vi "Main.vi"(11 "Module Admin":refnum<class "Delacor_lib_QMH_Cloneable Module Admin.lvclass">) -> ()   [LabVIEW 2020, in "Data Viewer.lvlib"]
doc: "This template is based off of the Queued Message Handler design pattern and the Queued Message Handler project template that ships with LabVIEW.\n\nThe main difference is that the queue is private to this module and communication between modules is performed via Broadcast and Request events.\n\nRequest events are wrapped in public API methods and are handled in the Event Handling Loop (EHL) of this VI. Any module can register for Broadcast events sent by this module. The EHL generates messages based on user interface actions.\n\nThe Message Handling Loop (MHL) processes messages generated by the EHL, or by other messages. The messages are string values, so new messages can be added easily to the Message Cases case structure in the MHL. Each message cluster can also provide an optional value for Message Data, which is a variant that can be converted to whatever message-specific data is required.\n_____\nBased on DQMH Project Template 7.0.1.1316."
uses:
  Data Viewer.lvlib
  <vilib>/Delacor/Delacor QMH/Libraries/Cloneable Module Admin_class/Delacor_lib_QMH_Cloneable Module Admin.lvclass
  C:/Program Files (x86)/National Instruments/LabVIEW 2020/vi.lib/Delacor/Delacor QMH/Libraries/Module Admin_class/Delacor_lib_QMH_Module Admin.lvclass
  Data Viewer/Legend.ctl
  Data Viewer/Filter Arguments.ctl
  Data Viewer/Filter Type.ctl
  Data Viewer/Filter Method.ctl
  <vilib>/Utility/miscctls.llb/LVPoint32TypeDef.ctl
  Data Viewer/Data Viewer.lvclass
  Data Viewer/Control Reference.ctl
  <vilib>/Delacor/Delacor QMH/Libraries/Cloneable Module Admin_class/Delacor_lib_QMH_Cloneable Module Admin.lvclass/Delacor_lib_QMH_Cloneable Module Admin.ctl
  <vilib>/Delacor/Delacor QMH/Libraries/Message Queue_class/Delacor_lib_QMH_Message Queue.lvclass/Delacor_lib_QMH_Message Queue.ctl
  Draw Plot Argument--cluster.ctl
  Filte Data Argument--cluster.ctl
  Menu Action Argument--cluster.ctl
  Open File Argument--cluster.ctl
  Restore Data Argument--cluster.ctl
  Set YScale Argument--cluster.ctl
  Show Value Argument--cluster.ctl
  Update Curve Color Argument--cluster.ctl
  Update Filter Arguments Argument--cluster.ctl
  Window Resize Argument--cluster.ctl
  Stop Argument--cluster.ctl
  Cut Half Data Argument--cluster.ctl
  Scale List Menu Action Argument--cluster.ctl
  Update Scale List Argument--cluster.ctl
  Initialize Plot List Argument--cluster.ctl
  Load Plot Argument--cluster.ctl
  Unload Plot Argument--cluster.ctl
  Show Hide Scale Argument--cluster.ctl
  Add Default Scale Argument--cluster.ctl
  Update Plot List Argument--cluster.ctl
  Add Virtual Cruve Argument--cluster.ctl
  Edit Curve Argument--cluster.ctl
  <vilib>/Utility/miscctls.llb/LVRectTypeDef.ctl
  <vilib>/Delacor/Delacor QMH/Libraries/Module Admin_class/Delacor_lib_QMH_Module Admin.lvclass/Delacor_lib_QMH_Module Admin.ctl
  Data Viewer/Scale Setting--cluster.ctl
  <vilib>/Delacor/Delacor QMH/Libraries/Cloneable Module Admin_class/Delacor_lib_QMH_Get Module ID.vi
  <vilib>/Delacor/Delacor QMH/Libraries/Message Queue_class/Delacor_lib_QMH_Enqueue Message (Single).vi
  <vilib>/Delacor/Delacor QMH/Libraries/Module Admin_class/Delacor_lib_QMH_Get External Launch.vi
  <vilib>/Delacor/Delacor QMH/Libraries/Message Queue_class/Delacor_lib_QMH_Message Queue.lvclass
panel:
  out "图例":T1
  out "Coords":T2
  in  "restore":bool
  in  "Open File":bool
  out "Plot List Select Index":i32
  in  "filter":bool
  in  "滤波参数":T3={"滤波器类型"=enum."Butterworth滤波器", "滤波方式"=enum."低通", "参数1"=1.0, "参数2"=1.0} {"参数2" format="%.2f"; "参数1" format="%.2f"}
  in  "half":bool
  out "Scale List Select Index":i32
  out "移动显示":string
  out "错误输出":errorcluster
  in  "选项卡控件":enum32{"选项卡 1"}(tab)
  in  "Add Virtual Curve":bool
  in  "坐标轴列表":i32(listbox) caption="Y坐标轴"
  in  "Filter Pane":enum32{"选项卡 1", "选项卡 2"}(tab)
  in  "Draw Plot":bool
  in  "X坐标轴":T6
  in  "曲线列表":T7(array[cluster]) caption="曲线" {"Scale" items=["温度", "湿度"]}
  in  "Simulate EHL Error":bool
  in  "Simulate MHL Error":bool
  out "XY图":cluster{"Time":timestamp[], "Value":dbl[]}[](graph)
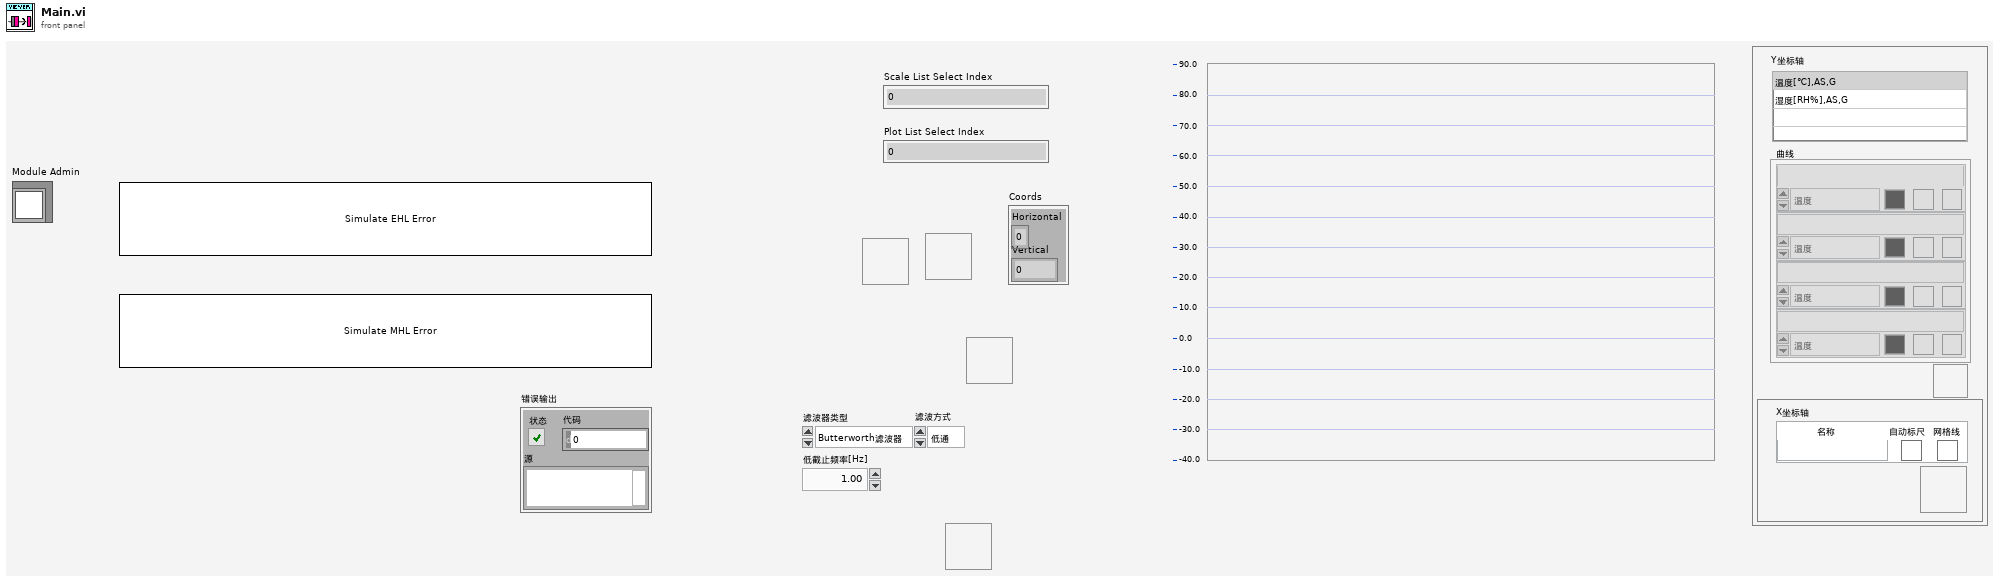
[diagram p1: front panel]
types:
  T1 = typedef "Data Viewer.lvlib/Data Viewer.lvclass/Legend.ctl" = cluster{"颜色":u32, "曲线名称":string}[]
  T2 = typedef "LVPoint32TypeDef.ctl" = cluster{"Horizontal":i32, "Vertical":i32}
  T3 = typedef "Data Viewer.lvlib/Data Viewer.lvclass/Filter Arguments.ctl" = cluster{"滤波器类型":T4, "滤波方式":T5, "参数1":dbl, "参数2":dbl}
  T4 = typedef "Data Viewer.lvlib/Data Viewer.lvclass/Filter Type.ctl" = enum16{"Butterworth滤波器", "中值滤波器"}
  T5 = typedef "Data Viewer.lvlib/Data Viewer.lvclass/Filter Method.ctl" = enum16{"低通", "高通", "带通", "带阻"}
  T6 = cluster{"名称":string, "Auto Scale":bool, "Gird Line":bool}
  T7 = cluster{"Name":string, "Scale":u16, "Color":u32, "Visible":bool, "Peak Line":bool}[]
  T8 = enum8{"Enabled", "Disabled", "Disabled and Grayed Out"}
  T9 = typedef "Data Viewer.lvlib/Data Viewer.lvclass/Control Reference.ctl" = cluster{"rVI":refnum<vi>, "r窗格":refnum<vi>, "rXY图":refnum<vi>, "r选项卡控件":refnum<vi>, "r图例":refnum<vi>, "r移动显示":refnum<vi>, "r滤波参数":refnum<vi>, "rFilter Pane ":refnum<vi>, "r坐标轴列表":refnum<vi>, "rAdd按钮":refnum<vi>, "r曲线列表":refnum<vi>}
  T10 = typedef "Data Viewer.lvlib/Request Events--cluster.ctl" = cluster{"Stop Module":refnum<user-event>, "Show Panel":refnum<user-event>, "Hide Panel":refnum<user-event>, "Show Diagram":refnum<user-event>, "Get Module Execution Status":refnum<user-event>, "Private":cluster{"Window Resize":refnum<user-event>, "Open File":refnum<user-event>, "Draw Plot":refnum<user-event>, "Set YScale":refnum<user-event>, "Update Curve Color":refnum<user-event>, "Show Value":refnum<user-event>, "Menu Action":refnum<user-event>, "Update Filter Arguments":refnum<user-event>, "Filte Data":refnum<user-event>, "Restore Data":refnum<user-event>, "Cut Half Data":refnum<user-event>, "Select Point":refnum<user-event>, "Open Linear Measurement":refnum<user-event>, "Linear Measurement Close":refnum<user-event>}, "Scale List Menu Action":refnum<user-event>, "Private.Update Scale List":refnum<user-event>, "Private.Initialize Plot List":refnum<user-event>, "Private.Load Plot":refnum<user-event>, "Private.Unload Plot":refnum<user-event>, "Show Hide Scale":refnum<user-event>, "Private.Add Default Scale":refnum<user-event>, "Private.Update Plot List":refnum<user-event>, "Private.Add Virtual Cruve":refnum<user-event>, "Private.Edit Curve":refnum<user-event>}
  T11 = typedef "Data Viewer.lvlib/Draw Plot Argument--cluster.ctl" = cluster{"Module ID":i32, "布尔":bool}
  T12 = typedef "Data Viewer.lvlib/Filte Data Argument--cluster.ctl" = cluster{"Module ID":i32, "布尔":bool}
  T13 = typedef "Data Viewer.lvlib/Menu Action Argument--cluster.ctl" = cluster{"Module ID":i32, "项标识符":string}
  T14 = typedef "Data Viewer.lvlib/Open File Argument--cluster.ctl" = cluster{"Module ID":i32, "布尔":bool}
  T15 = typedef "Data Viewer.lvlib/Restore Data Argument--cluster.ctl" = cluster{"Module ID":i32, "布尔":bool}
  T16 = typedef "Data Viewer.lvlib/Set YScale Argument--cluster.ctl" = cluster{"Module ID":i32, "布尔":bool}
  T17 = typedef "Data Viewer.lvlib/Show Value Argument--cluster.ctl" = cluster{"Module ID":i32, "坐标":T2}
  T18 = typedef "Data Viewer.lvlib/Update Curve Color Argument--cluster.ctl" = cluster{"Module ID":i32, "布尔":bool}
  T19 = typedef "Data Viewer.lvlib/Update Filter Arguments Argument--cluster.ctl" = cluster{"Module ID":i32, "布尔":bool}
  T20 = typedef "Data Viewer.lvlib/Window Resize Argument--cluster.ctl" = cluster{"Module ID":i32, "布尔":bool}
  T21 = enum32{"invalid lock state", "Not Locked", "Locked (No Password)", "Password-protected"}
  T22 = typedef "Data Viewer.lvlib/Stop Argument--cluster.ctl" = cluster{"Module ID":i32, "Origin":string, "Exit via Stop Module Req?":bool, "Wait for Module to stop?":bool}
  T23 = typedef "Data Viewer.lvlib/Cut Half Data Argument--cluster.ctl" = cluster{"Module ID":i32, "布尔":bool}
  T24 = typedef "Data Viewer.lvlib/Scale List Menu Action Argument--cluster.ctl" = cluster{"Module ID":i32, "ItemTag ":string, "Scale Index":i32}
  T25 = typedef "Data Viewer.lvlib/Update Scale List Argument--cluster.ctl" = cluster{"Module ID":i32, "Boolean":bool}
  T26 = typedef "Data Viewer.lvlib/Initialize Plot List Argument--cluster.ctl" = cluster{"Module ID":i32, "Boolean":bool}
  T27 = typedef "Data Viewer.lvlib/Load Plot Argument--cluster.ctl" = cluster{"Module ID":i32, "Plot Index":i32}
  T28 = typedef "Data Viewer.lvlib/Unload Plot Argument--cluster.ctl" = cluster{"Module ID":i32, "Plot Index":i32}
  T29 = typedef "Data Viewer.lvlib/Show Hide Scale Argument--cluster.ctl" = cluster{"Module ID":i32, "Scale Index":i32, "Visible":bool}
  T30 = typedef "Data Viewer.lvlib/Add Default Scale Argument--cluster.ctl" = cluster{"Module ID":i32, "Boolean":bool}
  T31 = typedef "Data Viewer.lvlib/Update Plot List Argument--cluster.ctl" = cluster{"Module ID":i32, "曲线列表":cluster{"Name":string, "Scale":u16, "Color":u32, "Visible":bool, "Peak Line":bool}[]}
  T32 = typedef "Data Viewer.lvlib/Add Virtual Cruve Argument--cluster.ctl" = cluster{"Module ID":i32, "Boolean":bool}
  T33 = typedef "Data Viewer.lvlib/Edit Curve Argument--cluster.ctl" = cluster{"Module ID":i32, "Plot Index":i32}
  T34 = typedef "LVRectTypeDef.ctl" = cluster{"Left":i16, "Top":i16, "Right":i16, "Bottom":i16}
  T35 = enum32{"Invalid", "Standard", "Closed", "Hidden", "Minimized", "Maximized"}
  T36 = cluster{"Name":string, "Scale":u16, "Color":u32, "Visible":bool, "Peak LIne":bool}
  T37 = cluster{"Name":string, "Scale":u16, "Color":u32, "Visible":bool, "Peak Line":bool}
  T38 = typedef "Data Viewer.lvlib/Data Viewer.lvclass/Scale Setting--cluster.ctl" = cluster{"Name":string, "Unit":string, "Color":u32, "Auto Scale":bool, "Scale Min":dbl, "Scale Max":dbl, "Scale Interval":dbl, "Show Gird":bool, "Log":bool}
  T39 = enum32{"invalid app kind", "Development System", "Run Time System", "Student Edition", "Embedded LabVIEW", "Evaluation", "Custom"}
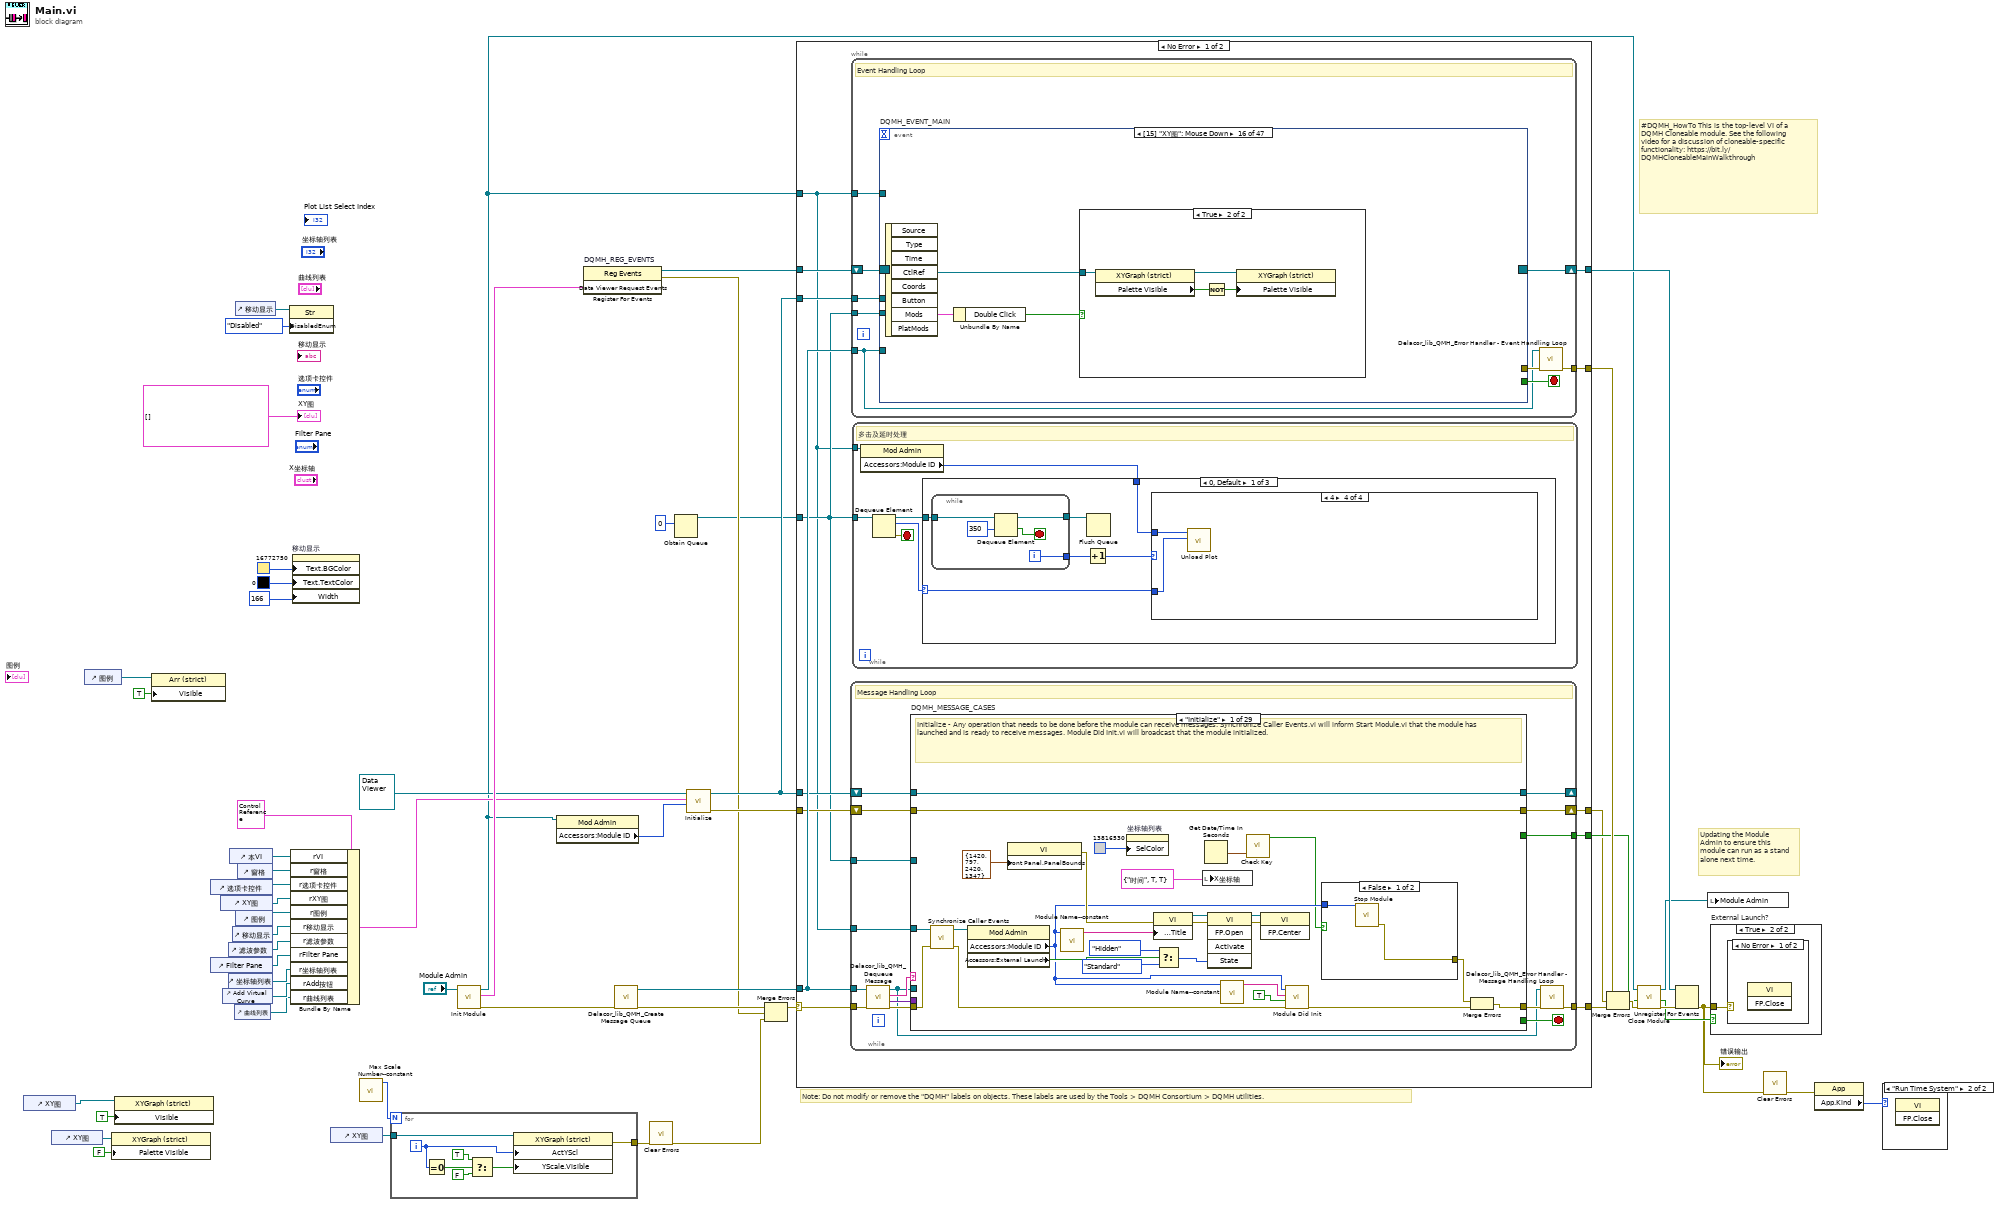
[diagram p0: block diagram]
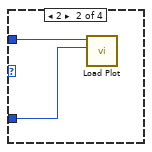
[diagram p4: hidden frame]
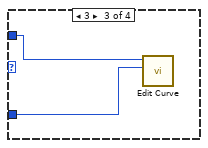
[diagram p5: hidden frame]
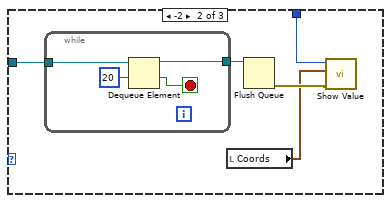
[diagram p6: hidden frame]
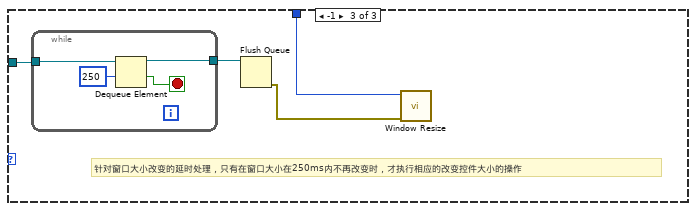
[diagram p7: hidden frame]
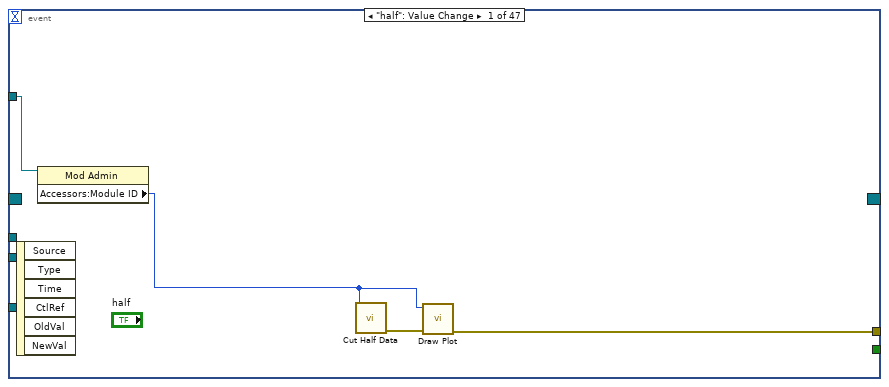
[diagram p8: hidden frame]
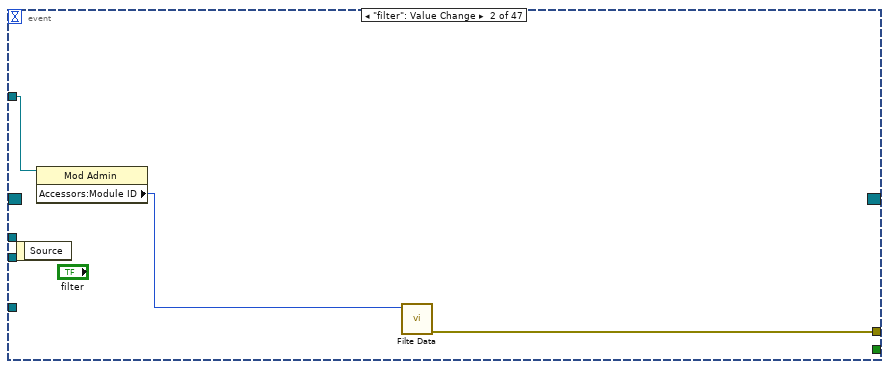
[diagram p9: hidden frame]
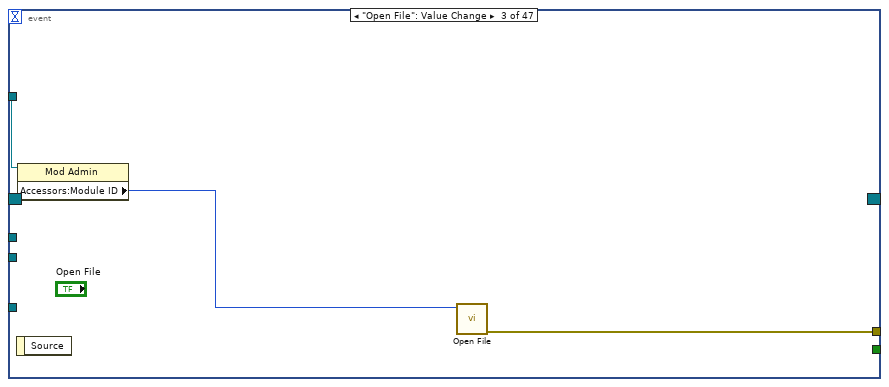
[diagram p10: hidden frame]
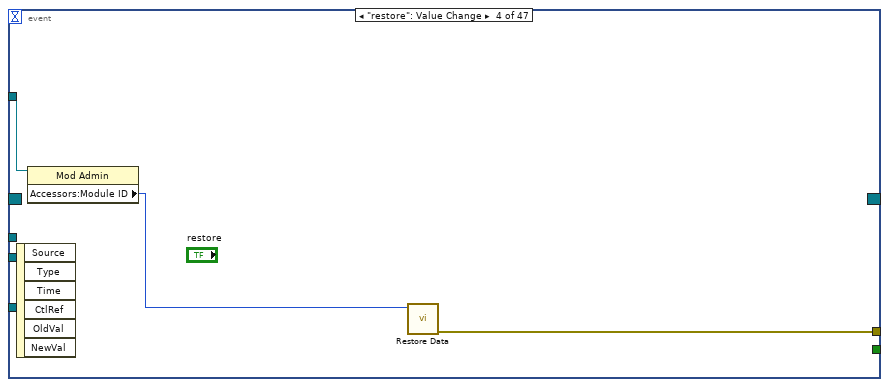
[diagram p11: hidden frame]
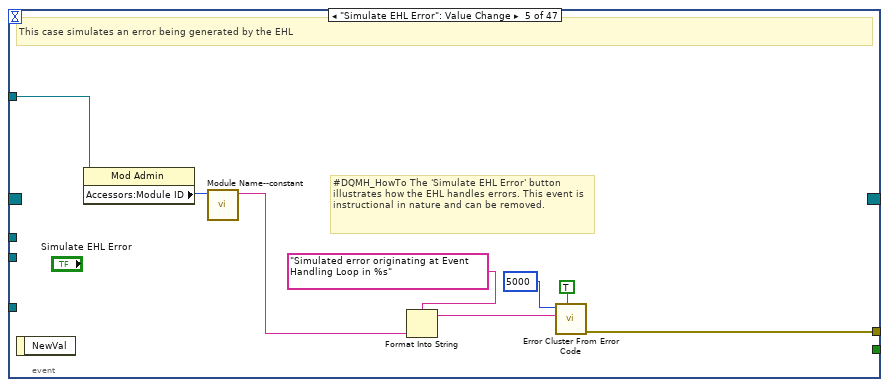
[diagram p12: hidden frame]
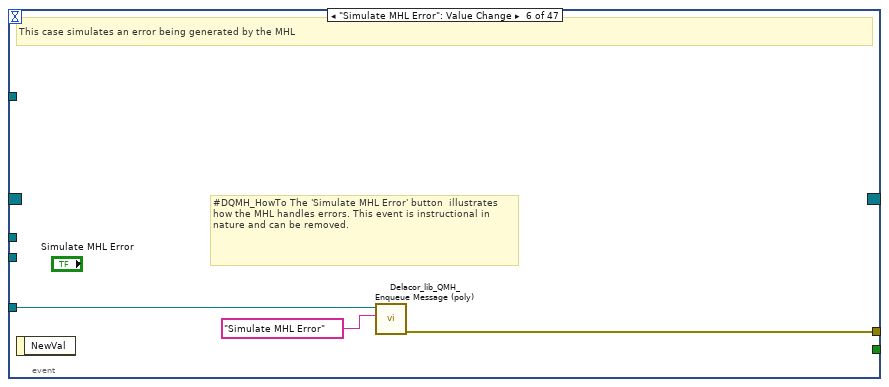
[diagram p13: hidden frame]
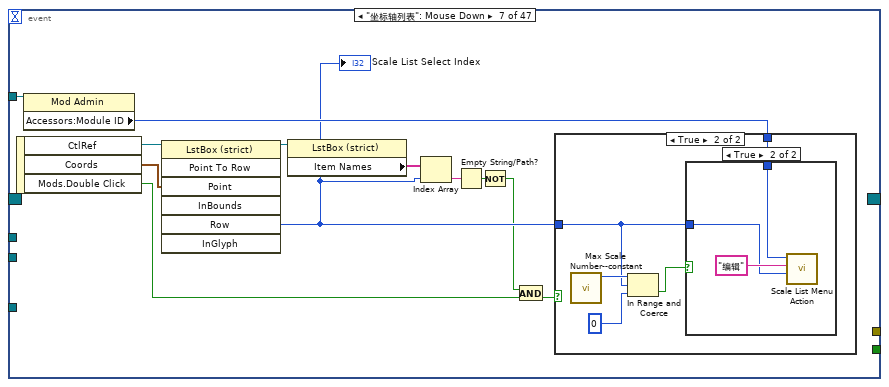
[diagram p14: hidden frame]
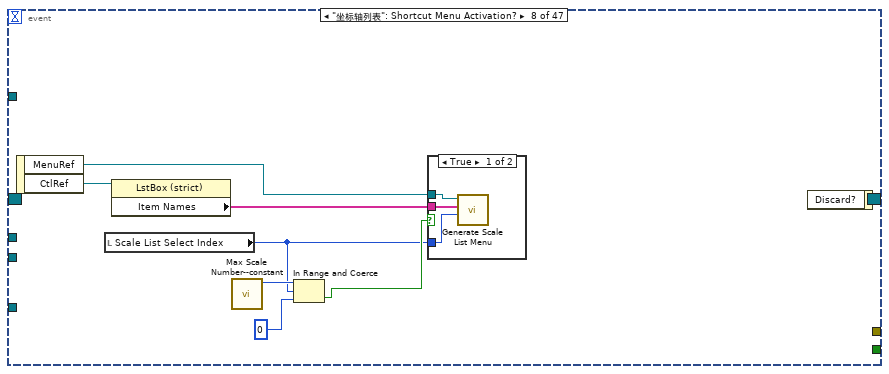
[diagram p17: hidden frame]
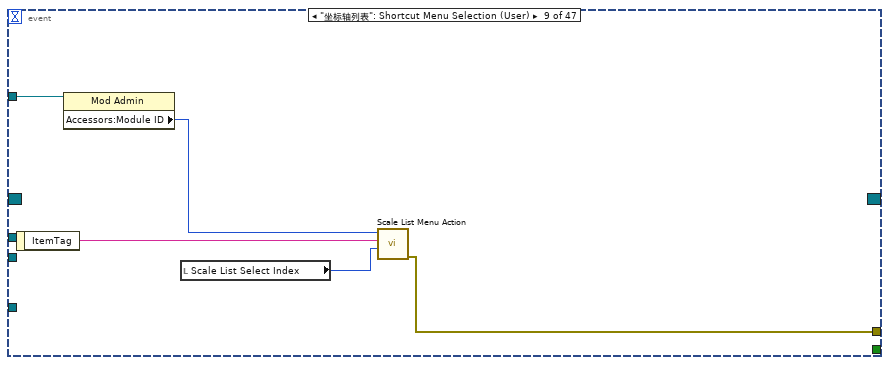
[diagram p19: hidden frame]
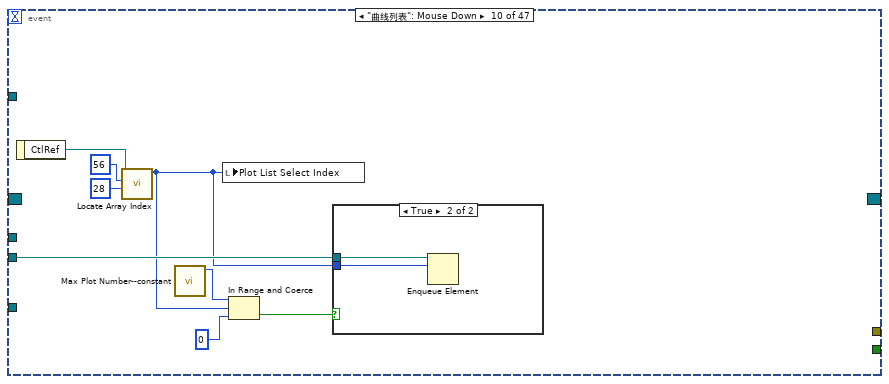
[diagram p20: hidden frame]
diagram:
  # "#DQMH_HowTo This is the top-level VI of a DQMH Cloneable module. See the following video for a discussion of cloneable-specific functionality: https://bit.ly/DQMHCloneableMainWalkthrough"
  # "Note: Do not modify or remove the \"DQMH\" labels on objects. These labels are used by the Tools > DQMH Consortium > DQMH utilities."
  # "Updating the Module Admin to ensure this module can run as a stand alone next time."
  n1 = control-ref of="XY图"() -> (w18:refnum<vi>)
  n2 = control-ref of="XY图"() -> (w2:refnum<vi>)
  n3 = control-ref of="图例"() -> (w4:refnum<vi>)
  n4 = property class="XYGraph (strict)"(reference=w2, "Palette Visible"=FALSE ("Palette:Visible")) -> ()  [unwired: 1 in, 2 out]
  n5 = property class="XYGraph (strict)"(reference=w18, "Visible"=TRUE) -> ()  [unwired: 1 in, 2 out]
  n6 = property class="Arr (strict)"(reference=w4, "Visible"=TRUE) -> ()  [unwired: 1 in, 2 out]
  n7 = control-ref of="选项卡控件"() -> (w34:refnum<vi>)
  n8 = control-ref of="Filter Pane"() -> (w30:refnum<vi>)
  n9 = control-ref of="XY图"() -> (w13:refnum<vi>)
  n10 = control-ref of="Add Virtual Curve"() -> (w6:refnum<vi>)
  n11 = control-ref of="滤波参数"() -> (w29:refnum<vi>)
  n12 = control-ref of="坐标轴列表"() -> (w23:refnum<vi>)
  n13 = control-ref of="本VI"() -> (w37:refnum<vi>)
  n14 = control-ref of="移动显示"() -> (w32:refnum<vi>)
  n15 = control-ref of="曲线列表"() -> (w5:refnum<vi>)
  n16 = control-ref of="移动显示"() -> (w28:refnum<vi>)
  n17 = control-ref of="图例"() -> (w33:refnum<vi>)
  n18 = control-ref of="窗格"() -> (w36:refnum<vi>)
  n19 = property class="Str"(reference=w28, "DisabledEnum"=T8."Disabled" ("禁用")) -> ()  [unwired: 1 in, 2 out]
  n20 = Bundle By Name(cluster=T9 {"rVI"=refnum, "r窗格"=refnum, "rXY图"=refnum, "r选项卡控件"=refnum, "r图例"=refnum, "r移动显示"=refnum, "r滤波参数"=refnum, "rFilter Pane "=refnum, "r坐标轴列表"=refnum, "rAdd按钮"=refnum, "r曲线列表"=refnum} ("Reference"), "rVI"=w37, "r窗格"=w36, "r选项卡控件"=w34, "rXY图"=w13, "r图例"=w33, "r移动显示"=w32, "r滤波参数"=w29, "rFilter Pane"=w30, "r坐标轴列表"=w23, "rAdd按钮"=w6, "r曲线列表"=w5) -> (w38:T9)
  n21 = property on="移动显示" class="Str"("Text.BGColor"=u32 16772750 ("Text.Text Colors:BG Color"), "Text.TextColor"=u32 0 ("Text.Text Colors:Text Color"), "Width"=u32 166 ("Size:Width")) -> ()  [unwired: 2 in, 2 out]
  n22 = control-ref of="XY图"() -> (w19:refnum<vi>)
  n23 = call "Max Scale Number--constant.vi"() -> ("Max Scale Number"=w20:i32)  [unwired: 11 in]
  n24 = for {
    N: w20 -> [_]
    tunnel: w19 -> [w63]
    tunnel: [w58] -> w16
    i -> [w62]
    n25 = Equal To 0?(x=w62) -> (x = 0?=w61:bool)
    n26 = Select(t=TRUE ("Visible"), s=w61, f=FALSE ("Visible")) -> (s? t:f=w57:bool)
    n27 = property class="XYGraph (strict)"(reference=w63, "ActYScl"=w62, "YScale.Visible"=w57) -> (error out=w58:errorcluster)  [unwired: 1 in, 1 out]
  }
  n28 = call "Init Module.vi"("Cloneable Module Admin in"="Module Admin") -> ("error out"=w53:errorcluster, "Data Viewer Request Events"=w47:T10, "Cloneable Module Admin out"=w25:refnum<class "Delacor_lib_QMH_Cloneable Module Admin.lvclass">)  [unwired: 7 in, 1 out]
  n29 = property class="Mod Admin"(reference=w25) -> ("Accessors:Module ID"=w24:i32)  [unwired: 1 in, 2 out]
  n30 = register-events "DQMH_REG_EVENTS"(w47) -> (reference out=w48:refnum<event-registration>, error out=w26:errorcluster)  [unwired: 2 in]
  n31 = call <vilib>:"Delacor_lib_QMH_Create Message Queue.vi"("error in"=w53) -> ("error out"=w51:errorcluster, "Message Queue"=w46:refnum<class "Delacor_lib_QMH_Message Queue.lvclass">)  [unwired: 9 in]
  n32 = call <vilib>:"Clear Errors.vi"("error in (no error)"=w16) -> ("error out"=w15:errorcluster)  [unwired: 5 in, 1 out]
  n33 = Obtain Queue(element data type=0) -> (queue out=w22:refnum<queue>)  [unwired: 4 in, 2 out]
  n34 = call "Initialize.vi"("Module ID"=w24, "Reference"=w38, "Data Viewer 输入"=refnum<class "Data Viewer.lvclass"> refnum ("DataSave.lvlib:Data Viewer.lvlib:Data Viewer.lvclass")) -> ("error out"=w40:errorcluster, "Data Viewer 输出"=w31:refnum<class "Data Viewer.lvclass">)  [unwired: 7 in]
  n35 = Merge Errors(w51, w26, w15) -> (w50:errorcluster)
  n36 = case shown="No Error" w50 {
    selector: w50 -> [w74 w947]
    tunnel: [w76 w946] -> w54
    tunnel: [w73 w945] -> w49
    tunnel: w48 -> [w72 w945]
    tunnel: w46 -> [w71 w938]
    tunnel: [w75 _] -> w55
    tunnel: w25 -> [w64 w941]
    tunnel: [w70 _] -> w43
    tunnel: w31 -> [w69 _]
    tunnel: w40 -> [w68 _]
    tunnel: [w67 _] -> w35
    tunnel: w31 -> [w66 _]
    tunnel: w22 -> [w65 _]
    frame No Error {
      n37 = while {
        tunnel: w71 -> [w557]
        shift-right: [w564] -> _
        shift-left: w69 -> [w565]
        tunnel: w74 -> [w568]
        tunnel: [w566] -> w76
        tunnel: w64 -> [w559]
        tunnel: [w558] -> w70
        shift-right: [w556] -> w67
        shift-left: w68 -> [w555]
        tunnel: w65 -> [w554]
        stop <- w563 stop-if-true
        # "Message Handling Loop"
        n38 = call-dynamic "Delacor_lib_QMH_Dequeue Message.vi"("error in"=w568, "Message Queue in"=w557) -> ("error out"=w567:errorcluster, "Message Data"=w561:variant, "Message"=w562:string, "Message Queue out"=w560:refnum<class "Delacor_lib_QMH_Message Queue.lvclass">)  [unwired: 6 in]
        n39 = case "DQMH_MESSAGE_CASES" shown="\"Initialize\"" w562 {
          selector: w562 -> [_ _ _ _ _ _ _ _ _ _ _ _ _ _ _ _ _ _ _ _ _ _ _ _ _ _ _ _ w927]
          tunnel: w560 -> [_ _ _ _ _ _ _ _ _ _ _ _ _ _ _ _ _ _ _ _ _ _ _ _ _ w875 _ w918 _]
          tunnel: w567 -> [w594 w606 w615 w628 w641 w650 w659 w669 w679 w688 w699 w709 w718 w730 w741 w762 w777 w804 w818 w830 w845 w854 w864 w868 w871 w884 w902 w924 w936]
          tunnel: [w578 w606 w614 w619 w632 w648 w658 w668 w678 w687 w698 w708 w717 w729 w740 w745 w776 w803 w816 w829 w844 w853 w863 w867 w871 w880 w901 w919 w937] -> w569
          tunnel: w565 -> [w582 w605 w610 w623 w640 w649 w654 w663 w674 w683 w694 w704 w711 w725 w736 w751 w772 w799 w817 w825 w840 w849 w859 w866 w870 w879 w899 w908 w934]
          tunnel: [w582 w605 w609 w621 w635 w644 w653 w662 w673 w682 w692 w700 w710 w724 w734 w749 w771 w798 w817 w824 w839 w847 w858 w866 w870 w879 w899 w906 w934] -> w564
          tunnel: [_ _ _ _ _ _ _ _ _ _ _ _ _ _ _ _ _ _ _ _ _ _ _ _ _ _ _ w917 _] -> w563
          tunnel: w561 -> [_ _ w613 w626 w638 w647 w657 w667 w677 w686 w697 w707 w716 w728 w739 w760 w775 w802 w815 w828 w843 w852 w862 _ _ w878 _ w915 _]
          tunnel: w559 -> [w584 _ _ _ _ _ _ _ _ _ _ _ _ _ _ _ _ _ _ _ _ _ _ _ _ w877 w897 w910 w933]
          tunnel: [_ _ _ _ _ _ _ _ _ _ _ _ _ _ _ _ _ _ _ _ _ _ _ _ _ _ _ w913 _] -> w558
          tunnel: [w581 w604 w607 w620 w630 w642 w651 w660 w672 w680 w689 w701 w712 w723 w733 w748 w769 w796 w812 w822 w837 w846 w856 w865 w869 w872 w891 w905 w925] -> w556
          tunnel: w555 -> [w581 w604 w608 w622 w634 w643 w652 w661 w671 w681 w691 w702 w713 w722 w735 w750 w770 w797 w812 w821 w838 w848 w857 w865 w869 w872 w891 w907 w925]
          tunnel: w554 -> [_ _ _ _ _ _ _ _ _ _ _ _ _ _ _ _ _ _ _ _ _ _ _ _ _ _ _ w904 _]
          frame "Initialize" {
            # "Initialize - Any operation that needs to be done before the module can receive messages. Synchronize Caller Events.vi will inform Start Module.vi that the module has launched and is ready to receive messages. Module Did Init.vi will broadcast that the module initialized."
            n40 = call "Synchronize Caller Events.vi"("error in"=w594, "Module Admin"=w584) -> ("error out"=w593:errorcluster, "Module Admin out"=w583:refnum<class "Delacor_lib_QMH_Cloneable Module Admin.lvclass">)  [unwired: 8 in]
            n41 = property on="Property Node" class="Mod Admin"(reference=w583) -> ("Accessors:Module ID"=w573:i32, "Accessors:External Launch"=w585:bool)  [unwired: 1 in, 2 out]
            n42 = property on="Property Node" class="VI"("Front Panel.PanelBounds"=T34 {"Left"=1420, "Top"=797, "Right"=2420, "Bottom"=1347} ("前面板窗口:前面板边界")) -> (error out=w576:errorcluster)  [unwired: 2 in, 1 out]
            n43 = call "Module Name--constant.vi"("Module ID"=w573) -> ("Module Name"=w580:string)  [unwired: 10 in]
            n44 = property on="坐标轴列表" class="LstBox (strict)"("SelColor"=u32 13816530 ("Selection Color")) -> ()  [unwired: 2 in, 2 out]
            n45 = property on="Property Node" class="VI"(error in=w576, "Front Panel.Title"=w580) -> (reference out=w592:refnum<vi>, error out=w596:errorcluster)  [unwired: 1 in]
            n46 = Select(t=T35."Hidden" ("State"), s=w585, f=T35."Standard" ("State")) -> (s? t:f=w588:T35)
            n47 = local write "X坐标轴"(T6 {"名称"="时间", "Auto Scale"=TRUE, "Gird Line"=TRUE} ("X坐标轴")) -> ()
            n48 = Get Date/Time In Seconds() -> (seconds since 1Jan1904=w570:timestamp)
            n49 = invoke on="Invoke Node" class="VI" method="FP.Open"(reference=w592, error in=w596, "State"=w588) -> (reference out=w591:refnum<vi>, error out=w595:errorcluster)  [unwired: 2 in, 3 out]
            n50 = call "Module Name--constant.vi"("Module ID"=w573) -> ("Module Name"=w586:string)  [unwired: 10 in]
            n51 = call "Check Key.vi"("current time"=w570) -> ("Valid?"=w571:bool)  [unwired: 10 in]
            n52 = invoke on="Invoke Node" class="VI" method="FP.Center"(reference=w591, error in=w595) -> ()  [unwired: 1 in, 3 out]
            n53 = call "Module Did Init.vi"("error in"=w593, "Initialized?"=TRUE, "Origin"=w586, "Module ID"=w573) -> ("error out"=w579:errorcluster)  [unwired: 7 in]
            n54 = case shown="False" w571 {
              tunnel: [w597 w600] -> w574
              tunnel: w573 -> [w598 w599]
              frame False {
                n55 = call "Stop Module.vi"("Module ID"=w598) -> ("error out"=w597:errorcluster)  [unwired: 10 in]
              }
              frame True {
                n56 = call "Update Filter Arguments.vi"("Module ID"=w599) -> ("error out"=w603:errorcluster)  [unwired: 10 in]
                n57 = call "Window Resize.vi"("error in"=w603, "Module ID"=w599) -> ("error out"=w602:errorcluster)  [unwired: 9 in]
                n58 = call "Initialize Plot List.vi"("error in"=w602, "Module ID"=w599) -> ("error out"=w601:errorcluster)  [unwired: 9 in]
                n59 = call "Add Default Scale.vi"("error in"=w601, "Module ID"=w599) -> ("error out"=w600:errorcluster)  [unwired: 9 in]
              }
            }
            n60 = Merge Errors(w574, w579) -> (w578:errorcluster)
          }
          frame "---Module Specific---" {
            # "Separator -- The following cases handle messages specific to this Module."
          }
          frame "Window Resize" {
            n61 = Variant To Data(error in=w615, type=T20 {"Module ID"=-1, "布尔"=FALSE} ("Window Resize Argument"), Variant=w613) -> (data=w611:T20, error out=w614:errorcluster)
            n62 = Unbundle By Name(w611) -> ()  [unwired: 2 out]
            n63 = call "Resize Panes.vi"("error in (no error)"=w608, "Data Viewer 输入"=w610) -> ("error out"=w607:errorcluster, "Data Viewer 输出"=w609:refnum<class "Data Viewer.lvclass">)  [unwired: 8 in]
          }
          frame "Open File" {
            n64 = Variant To Data(error in=w628, type=T14 {"Module ID"=-1, "布尔"=FALSE} ("Open File Argument"), Variant=w626) -> (data=w624:T14, error out=w627:errorcluster)
            n65 = Unbundle By Name(w624) -> ("Module ID"=w616:i32)  [unwired: 1 out]
            n66 = call "Set YScale.vi"("Module ID"=w616) -> ("error out"=w617:errorcluster)  [unwired: 10 in]
            n67 = call "Open File.vi"("error in (no error)"=w622, "Data Viewer 输入"=w623) -> ("error out"=w620:errorcluster, "Data Viewer 输出"=w621:refnum<class "Data Viewer.lvclass">)  [unwired: 8 in]
            n68 = call "Draw Plot.vi"("error in"=w617, "Module ID"=w616) -> ("error out"=w618:errorcluster)  [unwired: 9 in]
            n69 = Merge Errors(w618, w627) -> (w619:errorcluster)
          }
          frame "Draw Plot" {
            n70 = Variant To Data(error in=w641, type=T11 {"Module ID"=-1, "布尔"=FALSE} ("Draw Plot Argument"), Variant=w638) -> (data=w636:T11, error out=w639:errorcluster)
            n71 = Unbundle By Name(w636) -> ("Module ID"=w633:i32)  [unwired: 1 out]
            n72 = local read "X坐标轴"() -> (w629:T6)
            n73 = call "Draw Plot.vi"("error in (no error)"=w634, "X坐标轴"=w629, "Data Viewer 输入"=w640) -> ("error out"=w630:errorcluster, "Data Viewer 输出"=w635:refnum<class "Data Viewer.lvclass">)  [unwired: 7 in]
            n74 = call "Window Resize.vi"("error in"=w630, "Module ID"=w633) -> ("error out"=w631:errorcluster)  [unwired: 9 in]
            n75 = Merge Errors(w631, w639) -> (w632:errorcluster)
          }
          frame "Set YScale" {
            n76 = Variant To Data(error in=w650, type=T16 {"Module ID"=-1, "布尔"=FALSE} ("Set YScale Argument"), Variant=w647) -> (data=w645:T16, error out=w648:errorcluster)
            n77 = Unbundle By Name(w645) -> ()  [unwired: 2 out]
            n78 = call "Set YScale.vi"("error in (no error)"=w643, "Data Viewer 输入"=w649) -> ("error out"=w642:errorcluster, "Data Viewer 输出"=w644:refnum<class "Data Viewer.lvclass">)  [unwired: 8 in]
          }
          frame "Update Curve Color" {
            n79 = Variant To Data(error in=w659, type=T18 {"Module ID"=-1, "布尔"=FALSE} ("Update Curve Color Argument"), Variant=w657) -> (data=w655:T18, error out=w658:errorcluster)
            n80 = Unbundle By Name(w655) -> ()  [unwired: 2 out]
            n81 = call "Update Plot Color.vi"("error in (no error)"=w652, "Data Viewer 输入"=w654) -> ("error out"=w651:errorcluster, "Data Viewer 输出"=w653:refnum<class "Data Viewer.lvclass">)  [unwired: 8 in]
          }
          frame "Show Value" {
            n82 = Variant To Data(error in=w669, type=T17 {"Module ID"=-1, "坐标"={"Horizontal"=0, "Vertical"=0}} ("Show Value Argument"), Variant=w667) -> (data=w665:T17, error out=w668:errorcluster)
            n83 = Unbundle By Name(w665) -> ("坐标"=w664:T2)  [unwired: 1 out]
            n84 = call "Show Value.vi"("error in (no error)"=w661, "Coords"=w664, "Data Viewer 输入"=w663) -> ("error out"=w660:errorcluster, "Data Viewer 输出"=w662:refnum<class "Data Viewer.lvclass">)  [unwired: 6 in, 1 out]
          }
          frame "Menu Action" {
            n85 = Variant To Data(error in=w679, type=T13 {"Module ID"=-1, "项标识符"=""} ("Menu Action Argument"), Variant=w677) -> (data=w675:T13, error out=w678:errorcluster)
            n86 = Unbundle By Name(w675) -> ("项标识符"=w670:string)  [unwired: 1 out]
            n87 = call "Menu Action.vi"("error in (no error)"=w671, "项标识符"=w670, "Data Viewer 输入"=w674) -> ("error out"=w672:errorcluster, "Data Viewer 输出"=w673:refnum<class "Data Viewer.lvclass">)  [unwired: 7 in]
          }
          frame "Update Filter Arguments" {
            n88 = Variant To Data(error in=w688, type=T19 {"Module ID"=-1, "布尔"=FALSE} ("Update Filter Arguments Argument"), Variant=w686) -> (data=w684:T19, error out=w687:errorcluster)
            n89 = Unbundle By Name(w684) -> ()  [unwired: 2 out]
            n90 = call "Update Filter Arguments.vi"("error in (no error)"=w681, "Data Viewer 输入"=w683) -> ("error out"=w680:errorcluster, "Data Viewer 输出"=w682:refnum<class "Data Viewer.lvclass">)  [unwired: 8 in]
          }
          frame "Filte Data" {
            n91 = Variant To Data(error in=w699, type=T12 {"Module ID"=-1, "布尔"=FALSE} ("Filte Data Argument"), Variant=w697) -> (data=w695:T12, error out=w698:errorcluster)
            n92 = Unbundle By Name(w695) -> ()  [unwired: 2 out]
            n93 = call "Filte Data.vi"("error in (no error)"=w691, "Data Viewer 输入"=w694) -> ("error out"=w690:errorcluster, "Data Viewer 输出"=w693:refnum<class "Data Viewer.lvclass">)  [unwired: 8 in]
            n94 = call "Draw Plot.vi"("error in (no error)"=w690, "Data Viewer 输入"=w693) -> ("error out"=w689:errorcluster, "Data Viewer 输出"=w692:refnum<class "Data Viewer.lvclass">)  [unwired: 8 in]
          }
          frame "Restore Data" {
            n95 = Variant To Data(error in=w709, type=T15 {"Module ID"=-1, "布尔"=FALSE} ("Restore Data Argument"), Variant=w707) -> (data=w705:T15, error out=w708:errorcluster)
            n96 = Unbundle By Name(w705) -> ()  [unwired: 2 out]
            n97 = call "Restore Data.vi"("error in (no error)"=w702, "Data Viewer 输入"=w704) -> ("error out"=w701:errorcluster, "Data Viewer 输出"=w703:refnum<class "Data Viewer.lvclass">)  [unwired: 8 in]
            n98 = call "Draw Plot.vi"("Data Viewer 输入"=w703) -> ("Data Viewer 输出"=w700:refnum<class "Data Viewer.lvclass">)  [unwired: 9 in, 1 out]
          }
          frame "Cut Half Data" {
            n99 = Variant To Data(error in=w718, type=T23 {"Module ID"=-1, "布尔"=FALSE} ("Cut Half Data Argument"), Variant=w716) -> (data=w714:T23, error out=w717:errorcluster)
            n100 = Unbundle By Name(w714) -> ()  [unwired: 2 out]
            n101 = call "Cut Half Data.vi"("error in (no error)"=w713, "Data Viewer 输入"=w711) -> ("error out"=w712:errorcluster, "Data Viewer 输出"=w710:refnum<class "Data Viewer.lvclass">)  [unwired: 8 in]
          }
          frame "Scale List Menu Action" {
            n102 = Variant To Data(error in=w730, type=T24 {"Module ID"=-1, "ItemTag "="", "Scale Index"=0} ("Scale List Menu Action Argument"), Variant=w728) -> (data=w726:T24, error out=w729:errorcluster)
            n103 = Unbundle By Name(w726) -> ("Module ID"=w719:i32, "ItemTag"=w721:string, "Scale Index"=w720:i32)
            n104 = call "Scale List Menu Action.vi"("error in (no error)"=w722, "Scale Index"=w720, "ItemTag"=w721, "Data Viewer in"=w725) -> ("error out"=w723:errorcluster, "Data Viewer out"=w724:refnum<class "Data Viewer.lvclass">)  [unwired: 6 in]
            n105 = call "Update Scale List.vi"("Module ID"=w719) -> ()  [unwired: 10 in, 1 out]
          }
          frame "Update Scale List" {
            n106 = Variant To Data(error in=w741, type=T25 {"Module ID"=-1, "Boolean"=FALSE} ("Update Scale List Argument"), Variant=w739) -> (data=w737:T25, error out=w740:errorcluster)
            n107 = Unbundle By Name(w737) -> ()  [unwired: 2 out]
            n108 = call "Update Scale List.vi"("error in (no error)"=w735, "Data Viewer in"=w736) -> ("error out"=w733:errorcluster, "Scale Name List"=w731:string[], "Data Viewer out"=w734:refnum<class "Data Viewer.lvclass">)  [unwired: 7 in]
            n109 = control-ref of="Scale"() -> (w732:refnum<vi>)
            n110 = property class="Ring (strict)"(reference=w732, "Strings []"=w731) -> ()  [unwired: 1 in, 2 out]
          }
          frame "Initialize Plot List" {
            n111 = Variant To Data(error in=w762, type=T26 {"Module ID"=-1, "Boolean"=FALSE} ("Initialize Plot List Argument"), Variant=w760) -> (data=w743:T26, error out=w761:errorcluster)
            n112 = control-ref of="Scale"() -> (w758:refnum<vi>)
            n113 = Unbundle By Name(w743) -> ("Module ID"=w742:i32)
            n114 = property class="Ring (strict)"(reference=w758, "Strings []"=string[] []) -> ()  [unwired: 1 in, 2 out]
            n115 = call "Max Plot Number--constant.vi"() -> ("Numeric"=w756:i32)  [unwired: 11 in]
            n116 = for {
              N: w756 -> [_]
              tunnel: [w764] -> w746 mode=indexing
              tunnel: u32[] [16860, 16711680, 6665216, 15700480] -> [w763] mode=indexing
              n117 = Bundle By Name(cluster=T36 {"Name"="", "Scale"=0, "Color"=0, "Visible"=TRUE, "Peak LIne"=FALSE} ("Cluster"), "Color"=w763) -> (w764:T36)
            }
            n118 = local write "曲线列表"(w746) -> ()
            n119 = call "Initialize Plot Data.vi"("error in (no error)"=w750, "Data Viewer in"=w751) -> ("error out"=w748:errorcluster, "Data Viewer out"=w749:refnum<class "Data Viewer.lvclass">)  [unwired: 8 in]
            n120 = call "Update Plot List.vi"("曲线列表"=w746, "Module ID"=w742) -> ("error out"=w744:errorcluster)  [unwired: 9 in]
            n121 = Merge Errors(w744, w761) -> (w745:errorcluster)
            n122 = property on="Scale" class="Ring (strict)"("TipStrip"="选择坐标轴" ("Tip Strip")) -> ()  [unwired: 2 in, 2 out]
            n123 = property on="Color" class="ColBox"("TipStrip"="更改颜色" ("Tip Strip")) -> ()  [unwired: 2 in, 2 out]
            n124 = property on="Visible" class="Bool (strict)"("TipStrip"="显示/隐藏" ("Tip Strip")) -> ()  [unwired: 2 in, 2 out]
            n125 = property on="Peak Line" class="Bool (strict)"("TipStrip"="显示极值线" ("Tip Strip")) -> ()  [unwired: 2 in, 2 out]
          }
          frame "Load Plot" {
            n126 = Variant To Data(error in=w777, type=T27 {"Module ID"=-1, "Plot Index"=0} ("Load Plot Argument"), Variant=w775) -> (data=w773:T27, error out=w776:errorcluster)
            n127 = Unbundle By Name(w773) -> ("Plot Index"=w768:i32)  [unwired: 1 out]
            n128 = call "Load Plot.vi"("error in (no error)"=w770, "Plot Index"=w768, "Data Viewer in"=w772) -> ("error out"=w769:errorcluster, "Cancel?"=w766:bool, "Plot Name"=w767:string, "Data Viewer out"=w771:refnum<class "Data Viewer.lvclass">)  [unwired: 5 in]
            n129 = case shown="False" w766 {
              tunnel: w768 -> [w780 _]
              tunnel: w767 -> [w779 _]
              frame False {
                n130 = local read "曲线列表"() -> (w781:T7)
                n131 = in-place {
                  in-place-border: w779 -> [w783]
                  n132 = in-place-array #1(w781, w780) -> (w784:T37)
                  n133 = Bundle By Name(cluster=w784, "Name"=w783) -> (w782:T37)
                  n134 = in-place-array #1(w782) -> (w778:T7)  [unwired: 1 out]
                }
                n135 = local write "曲线列表"(w778) -> ()
              }
              frame True {
              }
            }
          }
          frame "Unload Plot" {
            n136 = Variant To Data(error in=w804, type=T28 {"Module ID"=-1, "Plot Index"=0} ("Unload Plot Argument"), Variant=w802) -> (data=w800:T28, error out=w803:errorcluster)
            n137 = Unbundle By Name(w800) -> ("Plot Index"=w795:i32, "Module ID"=w788:i32)
            n138 = local read "曲线列表"() -> (w794:T7)
            n139 = call "Unload Plot.vi"("error in (no error)"=w797, "Plot Index"=w795, "Data Viewer in"=w799) -> ("error out"=w796:errorcluster, "Data Viewer out"=w798:refnum<class "Data Viewer.lvclass">)  [unwired: 7 in]
            n140 = Index Array(array=w794, index=w795) -> (element=w793:T37)
            n141 = Unbundle By Name(w793) -> ("Color"=w786:u32, "Name"=w792:string)
            n142 = Bundle By Name(cluster=T37 {"Name"="", "Scale"=0, "Color"=0, "Visible"=TRUE, "Peak Line"=FALSE} ("new element/subarray"), "Color"=w786) -> (w785:T37)
            n143 = Empty String/Path?(string/path=w792) -> (empty?=w791:bool)
            n144 = Not(x=w791) -> (.not. x?=w790:bool)
            n145 = Replace Array Subset(array=w794, new element=w785, index=w795) -> (w789:T7)
            n146 = case shown="True" w790 {
              tunnel: w792 -> [_ w807]
              frame False {
              }
              frame True {
                n147 = Format Into String(format string="%s 已卸载！", initial string="曲线 ", w807) -> (resulting string=w805:string)  [unwired: 1 in, 1 out]
                n148 = One Button Dialog(message=w805) -> ()  [unwired: 1 in, 1 out]
              }
            }
            n149 = local write "曲线列表"(w789) -> ()
            n150 = call "Update Plot List.vi"("曲线列表"=w789, "Module ID"=w788) -> ()  [unwired: 9 in, 1 out]
          }
          frame "Show Hide Scale" {
            n151 = Variant To Data(error in=w818, type=T29 {"Module ID"=-1, "Scale Index"=0, "Visible"=FALSE} ("Show Hide Scale Argument"), Variant=w815) -> (data=w813:T29, error out=w816:errorcluster)
            n152 = Unbundle By Name(w813) -> ("Scale Index"=w810:i32, "Visible"=w809:bool)
            n153 = control-ref of="XY图"() -> (w811:refnum<vi>)
            n154 = property class="XYGraph (strict)"(reference=w811, "ActYScl"=w810, "YScale.Visible"=w809) -> ()  [unwired: 1 in, 2 out]
          }
          frame "Add Default Scale" {
            n155 = Variant To Data(error in=w830, type=T30 {"Module ID"=-1, "Boolean"=FALSE} ("Add Default Scale Argument"), Variant=w828) -> (data=w826:T30, error out=w829:errorcluster)
            n156 = Unbundle By Name(w826) -> ("Module ID"=w819:i32)  [unwired: 1 out]
            n157 = control-ref of="坐标轴列表"() -> (w823:refnum<vi>)
            n158 = for {
              tunnel: w823 -> [w833]
              shift-right: [w834] -> w824
              shift-left: w825 -> [w835]
              tunnel: [w832] -> w822
              tunnel: w821 -> [w832]
              tunnel: T38[] [{"Name"="温度", "Unit"="℃", "Color"=0, "Auto Scale"=TRUE, "Scale Min"=0.0, "Scale Max"=0.0, "Scale Interval"=0.0, "Show Gird"=TRUE, "Log"=FALSE}, {"Name"="湿度", "Unit"="RH%", "Color"=0, "Auto Scale"=TRUE, "Scale Min"=0.0, "Scale Max"=0.0, "Scale Interval"=0.0, "Show Gird"=TRUE, "Log"=FALSE}] -> [w831] mode=indexing
              n159 = call "Scale List Add Item.vi"("Sacle Setting Out"=w831, "r坐标轴列表"=w833, "Data Viewer in"=w835) -> ("Data Viewer out"=w834:refnum<class "Data Viewer.lvclass">)  [unwired: 8 in]
            }
            n160 = call "Update Scale List.vi"("Module ID"=w819) -> ()  [unwired: 10 in, 1 out]
          }
          frame "Update Plot List" {
            n161 = Variant To Data(error in=w845, type=T31 {"Module ID"=-1, "曲线列表"=[]} ("Update Plot List Argument"), Variant=w843) -> (data=w841:T31, error out=w844:errorcluster)
            n162 = Unbundle By Name(w841) -> ("曲线列表"=w836:T7)  [unwired: 1 out]
            n163 = call "Update Plot List.vi"("error in (no error)"=w838, "曲线列表"=w836, "Data Viewer in"=w840) -> ("error out"=w837:errorcluster, "Data Viewer out"=w839:refnum<class "Data Viewer.lvclass">)  [unwired: 7 in]
          }
          frame "Add Virtual Cruve" {
            n164 = Variant To Data(error in=w854, type=T32 {"Module ID"=-1, "Boolean"=FALSE} ("Add Virtual Cruve Argument"), Variant=w852) -> (data=w850:T32, error out=w853:errorcluster)
            n165 = Unbundle By Name(w850) -> ()  [unwired: 2 out]
            n166 = call "Add Virtual Curve.vi"("error in (no error)"=w848, "Data Viewer in"=w849) -> ("error out"=w846:errorcluster, "Data Viewer out"=w847:refnum<class "Data Viewer.lvclass">)  [unwired: 7 in, 1 out]
          }
          frame "Edit Curve" {
            n167 = Variant To Data(error in=w864, type=T33 {"Module ID"=-1, "Plot Index"=0} ("Edit Curve Argument"), Variant=w862) -> (data=w860:T33, error out=w863:errorcluster)
            n168 = Unbundle By Name(w860) -> ("Plot Index"=w855:i32)  [unwired: 1 out]
            n169 = call "Edit Curve.vi"("error in (no error)"=w857, "Plot Index"=w855, "Data Viewer in"=w859) -> ("error out"=w856:errorcluster, "Data Viewer out"=w858:refnum<class "Data Viewer.lvclass">)  [unwired: 6 in, 1 out]
          }
          frame "---Copy This Frame---" {
            # "Duplicate this frame when creating new messages.  Change this comment in the duplicated frame to describe this message."
            n170 = Merge Errors(w868) -> (w867:errorcluster)
          }
          frame "---Exit and Error Handling---" {
            # "Separator - the following cases handle errors and exit messages."
          }
          frame "Error" {
            # "#CodeRecommended - If the module is running in standalone mode (External Launch = FALSE), this code will pop up an error dialog and call the 'Exit' message if an error occurs. Add more fine-grained error management here."
            # "Error - Check the error message data and respond accordingly. This message is sent by the \"Error Handler\" VIs at the end of each loop in this application."
            n171 = property on="Property Node" class="Mod Admin"(reference=w877) -> ("Accessors:External Launch"=w876:bool, "Accessors:Module ID"=w874:i32)  [unwired: 1 in, 2 out]
            n172 = Variant To Data(error in=w884, type=errorcluster {"status"=FALSE, "code"=0, "source"=""} ("error constant"), Variant=w878) -> (data=w873:errorcluster, error out=w882:errorcluster)
            n173 = local write "错误输出"(w873) -> ()
            n174 = call "Error Reported.vi"("Error"=w873, "Module ID"=w874) -> ()  [unwired: 9 in, 1 out]
            n175 = case shown="False" w876 {
              tunnel: [w889 _] -> w881
              tunnel: w875 -> [w887 _]
              tunnel: w873 -> [w888 _]
              frame False {
                n176 = disable-structure shown="Default" {
                  disable-tunnel: w888 -> [w890 _]
                  frame condition #0 (active) {
                    # "If the module is running standalone, then pop up an error dialog and call the \"Exit\" message."
                    n177 = call <vilib>:"Simple Error Handler.vi"("error in (no error)"=w890) -> ()  [unwired: 4 in, 5 out]
                  }
                  frame condition #1 {
                    # "To prevent the Simple Error Handler VI from being loaded (e.g. when deploying to a Real-Time target), add the Conditional Disable Symbol \"DQMH_Disable_SEH\" to your project and set it to TRUE."
                  }
                }
                n178 = call-poly <vilib>:"Delacor_lib_QMH_Enqueue Message (poly).vi"("Priority Message? (F)"=TRUE, "Message"="Exit", "Message Queue in"=w887) -> ("error out"=w889:errorcluster)  [unwired: 7 in, 1 out]
              }
              frame True {
                # "If the module was launched externally, calling the Error Reported broadcast VI is the only action performed by the \"Error\" message. The module's caller can then process the error appropriately."
              }
            }
            n179 = Merge Errors(w882, w881) -> (w880:errorcluster)
          }
          frame "Simulate MHL Error" {
            # "#DQMH_HowTo The 'Simulate MHL Error' button  illustrates how the MHL handles errors. This event is instructional in nature and can be removed."
            # "Simulate an error occurring at the MHL"
            n180 = property on="Property Node" class="Mod Admin"(reference=w897) -> ("Accessors:Module ID"=w898:i32)  [unwired: 1 in, 2 out]
            n181 = call "Module Name--constant.vi"("Module ID"=w898) -> ("Module Name"=w893:string)  [unwired: 10 in]
            n182 = Format Into String(format string="Simulated error originating at Message Handling Loop in %s", w893) -> (resulting string=w894:string)  [unwired: 2 in, 1 out]
            n183 = call <vilib>:"Error Cluster From Error Code.vi"("show call chain? (False)"=TRUE, "error message (\"\")"=w894, "error code (0)"=5001) -> ("error out"=w900:errorcluster)  [unwired: 6 in]
            n184 = Merge Errors(w902, w900) -> (w901:errorcluster)
          }
          frame "Exit" {
            w916 = 91  # 91: not all Exit messages will have an argument
            w917 = TRUE  # Stop the VI
            # "Release the message queue reference"
            # "#CodeNeeded - Add any required cleanup code here."
            # "Exit - Exit the application."
            n185 = Variant To Data(error in=w924, type=T22 {"Module ID"=-1, "Origin"="", "Exit via Stop Module Req?"=FALSE, "Wait for Module to stop?"=FALSE} ("Stop Argument"), Variant=w915) -> (data=w912:T22, error out=w920:errorcluster)
            n186 = call <vilib>:"Clear Errors.vi"("error in (no error)"=w920, "specific error code to clear (0: all)"=w916) -> ("error out"=w923:errorcluster)  [unwired: 4 in, 1 out]
            n187 = property on="Property Node" class="Mod Admin"(reference=w910) -> ("Accessors:Module ID"=w909:i32)  [unwired: 1 in, 2 out]
            n188 = control-ref of="This VI"() -> (w911:refnum<vi>)
            n189 = call-dynamic "Delacor_lib_QMH_Release Message Queue.vi"("error in"=w923, "Message Queue"=w918) -> ("error out"=w922:errorcluster)  [unwired: 9 in]
            n190 = call "Handle Exit.vi"("Stop Argument"=w912, "Module Admin in"=w910, "VI reference"=w911) -> ("error out"=w921:errorcluster, "Wait for Stop?"=w913:bool)  [unwired: 7 in]
            n191 = Merge Errors(w922, w921) -> (w919:errorcluster)
            n192 = call "Exit.vi"("error in (no error)"=w907, "Data Viewer 输入"=w908) -> ("error out"=w905:errorcluster, "Data Viewer 输出"=w906:refnum<class "Data Viewer.lvclass">)  [unwired: 8 in]
            n193 = Release Queue(queue=w904) -> (error out=w903:errorcluster)  [unwired: 2 in, 2 out]
            n194 = call "Error Reported.vi"("Error"=w919, "Module ID"=w909) -> ()  [unwired: 9 in, 1 out]
            n195 = call <vilib>:"Clear Errors.vi"("error in (no error)"=w903) -> ()  [unwired: 5 in, 2 out]
          }
          frame Default {
            # "'Default' case only runs if there is a message that isn't defined in any of the other cases.  Output a programming error."
            n196 = property on="Property Node" class="Mod Admin"(reference=w933) -> ("Accessors:Module ID"=w932:i32)  [unwired: 1 in, 2 out]
            n197 = call "Module Name--constant.vi"("Module ID"=w932) -> ("Module Name"=w926:string)  [unwired: 10 in]
            n198 = Format Into String(format string="The invalid message string \"%s\" was received in the Message Handling Loop for module \"%s\".", w927, w926) -> (resulting string=w929:string)  [unwired: 2 in, 1 out]
            n199 = call <vilib>:"Error Cluster From Error Code.vi"("show call chain? (False)"=TRUE, "error message (\"\")"=w929, "error code (0)"=1) -> ("error out"=w935:errorcluster)  [unwired: 6 in]
            n200 = Merge Errors(w936, w935) -> (w937:errorcluster)
          }
        }
        n201 = call-dynamic "Delacor_lib_QMH_Error Handler - Message Handling Loop.vi"("error in"=w569, "Message Queue in"=w560) -> ("dup error in"=w566:errorcluster)  [unwired: 8 in, 1 out]
      }
      n202 = while {
        tunnel: w71 -> [w120]
        shift-right: [w122] -> w73
        shift-left: w72 -> [w123]
        tunnel: [w124] -> w75
        tunnel: w64 -> [w118]
        tunnel: w66 -> [w119]
        tunnel: w65 -> [w117]
        stop <- w121 stop-if-true
        # "Event Handling Loop"
        n203 = event "DQMH_EVENT_MAIN" shown="[15] \"XY图\": Mouse Down" {
          selector: w123 -> [_ _ _ _ _ _ _ _ _ _ _ _ _ _ _ _ _ _ _ _ _ _ _ _ _ _ _ _ _ _ _ _ _ _ _ _ _ _ _ _ _ _ _ _ _ _ _]
          dyn-events: [_ _ _ _ _ _ _ _ _ _ _ _ _ _ _ _ _ _ _ _ _ _ _ _ _ _ _ _ _ _ _ _ _ _ _ _ _ _ _ _ _ _ _ _ _ _ _] -> w122
          timeout: _ -> [_ _ _ _ _ _ _ _ _ _ _ _ _ _ _ _ _ _ _ _ _ _ _ _ _ _ _ _ _ _ _ _ _ _ _ _ _ _ _ _ _ _ _ _ _ _ _]
          tunnel: [_ _ _ _ _ _ _ _ _ _ _ _ _ _ _ _ _ _ _ _ _ _ _ _ _ _ _ _ _ _ _ _ _ w386 _ _ _ _ _ _ _ _ _ _ _ _ _] -> w121
          tunnel: w120 -> [_ _ _ _ _ w148 _ _ _ _ _ _ _ _ _ _ _ _ _ _ _ w247 w259 w271 w283 w295 w307 w319 w331 w343 w355 _ _ w389 _ w407 w427 w440 w452 w464 w476 w488 w501 w513 w525 w537 w549]
          tunnel: [w126 w130 w133 w136 w146 w149 _ _ w182 _ w196 w199 w202 w205 _ _ w219 w222 _ w229 _ w240 w252 w264 w276 w288 w300 w312 w324 w336 w348 _ _ w390 _ w410 w420 w432 w445 w457 w469 w481 w493 w506 w518 w530 w542] -> w125
          tunnel: w119 -> [_ _ _ _ _ _ _ _ _ _ _ _ w204 _ _ _ _ _ _ _ _ _ _ _ _ _ _ _ _ _ _ _ _ _ _ _ _ _ _ _ _ _ _ _ _ _ _]
          tunnel: w118 -> [w129 w132 w135 w138 w145 _ w158 _ w181 _ w198 w201 _ w208 _ _ w221 w224 w225 w227 w233 w245 w257 w269 w281 w293 w305 w317 w329 w341 w353 w360 w376 w388 _ w408 w425 w438 w450 w462 w474 w486 w499 w511 w523 w535 w547]
          tunnel: w117 -> [_ _ _ _ _ _ _ _ _ w189 _ _ _ _ w209 _ _ _ _ _ _ _ _ _ _ _ _ _ _ _ _ _ _ _ w404 _ _ _ _ _ _ _ _ _ _ _ _]
          event "half": Value Change {
            n204 = event-data() -> ()  [unwired: 1 in, 6 out]
            n205 = property class="Mod Admin"(reference=w129) -> ("Accessors:Module ID"=w127:i32)  [unwired: 1 in, 2 out]
            n206 = call "Cut Half Data.vi"("Module ID"=w127) -> ("error out"=w128:errorcluster)  [unwired: 10 in]
            n207 = call "Draw Plot.vi"("error in"=w128, "Module ID"=w127) -> ("error out"=w126:errorcluster)  [unwired: 9 in]
          }
          event "filter": Value Change {
            n208 = event-data() -> ()  [unwired: 1 in, 1 out]
            n209 = property class="Mod Admin"(reference=w132) -> ("Accessors:Module ID"=w131:i32)  [unwired: 1 in, 2 out]
            n210 = call "Filte Data.vi"("Module ID"=w131) -> ("error out"=w130:errorcluster)  [unwired: 10 in]
          }
          event "Open File": Value Change {
            n211 = event-data() -> ()  [unwired: 1 in, 1 out]
            n212 = property class="Mod Admin"(reference=w135) -> ("Accessors:Module ID"=w134:i32)  [unwired: 1 in, 2 out]
            n213 = call "Open File.vi"("Module ID"=w134) -> ("error out"=w133:errorcluster)  [unwired: 10 in]
          }
          event "restore": Value Change {
            n214 = event-data() -> ()  [unwired: 1 in, 6 out]
            n215 = property class="Mod Admin"(reference=w138) -> ("Accessors:Module ID"=w137:i32)  [unwired: 1 in, 2 out]
            n216 = call "Restore Data.vi"("Module ID"=w137) -> ("error out"=w136:errorcluster)  [unwired: 10 in]
          }
          event "Simulate EHL Error": Value Change {
            # "#DQMH_HowTo The 'Simulate EHL Error' button  illustrates how the EHL handles errors. This event is instructional in nature and can be removed."
            # "This case simulates an error being generated by the EHL"
            n217 = event-data() -> ()  [unwired: 1 in, 1 out]
            n218 = property on="Property Node" class="Mod Admin"(reference=w145) -> ("Accessors:Module ID"=w144:i32)  [unwired: 1 in, 2 out]
            n219 = call "Module Name--constant.vi"("Module ID"=w144) -> ("Module Name"=w139:string)  [unwired: 10 in]
            n220 = Format Into String(format string="Simulated error originating at Event Handling Loop in %s", w139) -> (resulting string=w142:string)  [unwired: 2 in, 1 out]
            n221 = call <vilib>:"Error Cluster From Error Code.vi"("show call chain? (False)"=TRUE, "error message (\"\")"=w142, "error code (0)"=5000) -> ("error out"=w146:errorcluster)  [unwired: 6 in]
          }
          event "Simulate MHL Error": Value Change {
            # "#DQMH_HowTo The 'Simulate MHL Error' button  illustrates how the MHL handles errors. This event is instructional in nature and can be removed."
            # "This case simulates an error being generated by the MHL"
            n222 = event-data() -> ()  [unwired: 1 in, 1 out]
            n223 = call-poly <vilib>:"Delacor_lib_QMH_Enqueue Message (poly).vi"("Message"="Simulate MHL Error", "Message Queue in"=w148) -> ("error out"=w149:errorcluster)  [unwired: 8 in, 1 out]
          }
          event "坐标轴列表": Mouse Down {
            n224 = event-data() -> ("CtlRef"=w161:refnum<vi>, "Coords"=w160:T2, "Mods.Double Click"=w159:bool)  [unwired: 1 in]
            n225 = property class="Mod Admin"(reference=w158) -> ("Accessors:Module ID"=w157:i32)  [unwired: 1 in, 2 out]
            n226 = invoke class="LstBox (strict)" method="Point To Row"(reference=w161, "Point"=w160) -> (reference out=w156:refnum<vi>, "Row"=w154:i32)  [unwired: 5 in, 5 out]
            "Scale List Select Index" <- w154
            n227 = property class="LstBox (strict)"(reference=w156) -> ("Item Names"=w155:string[])  [unwired: 1 in, 2 out]
            n228 = Index Array(array=w155, index=w154) -> (element=w153:string)
            n229 = Empty String/Path?(string/path=w153) -> (empty?=w152:bool)
            n230 = Not(x=w152) -> (.not. x?=w150:bool)
            n231 = And(x=w150, y=w159) -> (x .and. y?=w151:bool)
            n232 = case shown="True" w151 {
              tunnel: w154 -> [_ w163]
              tunnel: w157 -> [_ w162]
              frame False {
              }
              frame True {
                n233 = call "Max Scale Number--constant.vi"() -> ("Max Scale Number"=w166:i32)  [unwired: 11 in]
                n234 = In Range and Coerce(upper limit=w166, x=w163, lower limit=0) -> (In Range?=w164:bool)  [unwired: 1 out]
                n235 = case shown="True" w164 {
                  tunnel: w163 -> [_ w168]
                  tunnel: w162 -> [_ w167]
                  frame False {
                  }
                  frame True {
                    n236 = call "Scale List Menu Action.vi"("Scale Index"=w168, "ItemTag"="编辑", "Module ID"=w167) -> ()  [unwired: 8 in, 1 out]
                  }
                }
              }
            }
          }
          event "坐标轴列表": Shortcut Menu Activation? {
            n237 = event-data() -> ("MenuRef"=w176:refnum<k9>, "CtlRef"=w175:refnum<vi>)  [unwired: 1 in]
            n238 = local read "Scale List Select Index"() -> (w171:i32)
            n239 = property class="LstBox (strict)"(reference=w175) -> ("Item Names"=w174:string[])  [unwired: 1 in, 2 out]
            n240 = call "Max Scale Number--constant.vi"() -> ("Max Scale Number"=w173:i32)  [unwired: 11 in]
            n241 = In Range and Coerce(upper limit=w173, x=w171, lower limit=0) -> (In Range?=w172:bool)  [unwired: 1 out]
            n242 = case shown="True" w172 {
              tunnel: w176 -> [w179 _]
              tunnel: w174 -> [w178 _]
              tunnel: w171 -> [w177 _]
              frame True {
                n243 = call "Generate Scale List Menu.vi"("Scale List Select Index"=w177, "Item Names"=w178, "Menu in"=w179) -> ()  [unwired: 9 in]
              }
              frame False {
              }
            }
            n244 = event-data() -> ()  [unwired: 2 in, 1 out]
          }
          event "坐标轴列表": Shortcut Menu Selection (User) {
            n245 = event-data() -> ("ItemTag"=w184:string)  [unwired: 1 in]
            n246 = property class="Mod Admin"(reference=w181) -> ("Accessors:Module ID"=w180:i32)  [unwired: 1 in, 2 out]
            n247 = local read "Scale List Select Index"() -> (w183:i32)
            n248 = call "Scale List Menu Action.vi"("Scale Index"=w183, "ItemTag"=w184, "Module ID"=w180) -> ("error out"=w182:errorcluster)  [unwired: 8 in]
          }
          event "曲线列表": Mouse Down {
            n249 = event-data() -> ("CtlRef"=w190:refnum<vi>)  [unwired: 1 in]
            n250 = call "Locate Array Index.vi"("Top Height"=28 ("x"), "Row Height"=56, "Array in"=w190) -> ("Index"=w185:i32)  [unwired: 8 in]
            n251 = call "Max Plot Number--constant.vi"() -> ("Numeric"=w187:i32)  [unwired: 11 in]
            n252 = local write "Plot List Select Index"(w185) -> ()
            n253 = In Range and Coerce(upper limit=w187, x=w185, lower limit=0) -> (In Range?=w186:bool)  [unwired: 1 out]
            n254 = case shown="True" w186 {
              tunnel: w189 -> [_ w194]
              tunnel: w185 -> [_ w193]
              frame False {
              }
              frame True {
                n255 = Enqueue Element(queue=w194, element=w193) -> ()  [unwired: 2 in, 3 out]
              }
            }
          }
          event "曲线列表": Value Change {
            n256 = event-data() -> ("NewVal"=w195:T7)  [unwired: 1 in, 5 out]
            n257 = property class="Mod Admin"(reference=w198) -> ("Accessors:Module ID"=w197:i32)  [unwired: 1 in, 2 out]
            n258 = call "Update Plot List.vi"("曲线列表"=w195, "Module ID"=w197) -> ("error out"=w196:errorcluster)  [unwired: 9 in]
          }
          event "Draw Plot": Value Change {
            n259 = event-data() -> ()  [unwired: 1 in, 6 out]
            n260 = property class="Mod Admin"(reference=w201) -> ("Accessors:Module ID"=w200:i32)  [unwired: 1 in, 2 out]
            n261 = call "Draw Plot.vi"("Module ID"=w200) -> ("error out"=w199:errorcluster)  [unwired: 10 in]
          }
          event "XY图": Shortcut Menu Activation? {
            n262 = event-data() -> ("MenuRef"=w203:refnum<k9>)  [unwired: 1 in]
            n263 = call "Genertate Menu.vi"("菜单引用"=w203, "Data Viewer 输入"=w204) -> ("error out"=w202:errorcluster)  [unwired: 8 in, 1 out]
            n264 = event-data() -> ()  [unwired: 2 in, 1 out]
          }
          event "XY图": Shortcut Menu Selection (User) {
            n265 = event-data() -> ("ItemTag"=w206:string)  [unwired: 1 in]
            n266 = property class="Mod Admin"(reference=w208) -> ("Accessors:Module ID"=w207:i32)  [unwired: 1 in, 2 out]
            n267 = call "Menu Action.vi"("项标识符"=w206, "Module ID"=w207) -> ("error out"=w205:errorcluster)  [unwired: 9 in]
          }
          event "XY图": Mouse Move {
            n268 = event-data() -> ("Coords"=→"Coords":T2)  [unwired: 1 in]
            n269 = Enqueue Element(queue=w209, element=-2) -> ()  [unwired: 2 in, 3 out]
          }
          event "XY图": Mouse Down {
            n270 = event-data() -> ("CtlRef"=w212:refnum<vi>, "Mods"=w214:cluster{"Double Click":bool, "Menu Key":bool})  [unwired: 1 in, 6 out]
            n271 = Unbundle By Name(w214) -> ("Double Click"=w213:bool)
            n272 = case shown="True" w213 {
              tunnel: w212 -> [_ w218]
              frame False {
              }
              frame True {
                n273 = property class="XYGraph (strict)"(reference=w218) -> (reference out=w217:refnum<vi>, "Palette Visible"=w216:bool)  [unwired: 1 in, 1 out]
                n274 = Not(x=w216) -> (.not. x?=w215:bool)
                n275 = property class="XYGraph (strict)"(reference=w217, "Palette Visible"=w215) -> ()  [unwired: 1 in, 2 out]
              }
            }
          }
          event "Add Virtual Curve": Value Change {
            n276 = event-data() -> ()  [unwired: 1 in, 6 out]
            n277 = property class="Mod Admin"(reference=w221) -> ("Accessors:Module ID"=w220:i32)  [unwired: 1 in, 2 out]
            n278 = call "Add Virtual Cruve.vi"("Module ID"=w220) -> ("error out"=w219:errorcluster)  [unwired: 10 in]
          }
          event Value Change {
            n279 = event-data() -> ()  [unwired: 1 in, 1 out]
            n280 = property class="Mod Admin"(reference=w224) -> ("Accessors:Module ID"=w223:i32)  [unwired: 1 in, 2 out]
            n281 = call "Update Filter Arguments.vi"("Module ID"=w223) -> ("error out"=w222:errorcluster)  [unwired: 10 in]
          }
          event Value Change {
            n282 = event-data() -> ()  [unwired: 1 in, 1 out]
            n283 = property class="Mod Admin" props=["Accessors:Module ID"](reference=w225) -> ()  [unwired: 1 in, 3 out]
          }
          event User Event {
            # "For cloneable running as singleton, broadcast that the module is running."
            n284 = event-data() -> ("Module ID"=w226:i32)  [unwired: 1 in]
            n285 = call "Addressed to This Module.vi"("Module ID from Argument"=w226, "Module Admin"=w227) -> ("Addressed to this instance?"=w228:bool)  [unwired: 8 in, 1 out]
            n286 = case shown="True" w228 {
              tunnel: [_ w232] -> w229
              tunnel: w226 -> [_ w231]
              frame False {
              }
              frame True {
                n287 = call "Update Module Execution Status.vi"("Running?"=TRUE, "Module ID"=w231) -> ("error out"=w232:errorcluster)  [unwired: 9 in]
              }
            }
          }
          event User Event {
            # "Another Module called the \"Hide Panel\" API Method."
            n288 = event-data() -> ("Module ID"=w234:i32)  [unwired: 1 in]
            n289 = call "Addressed to This Module.vi"("Module ID from Argument"=w234, "Module Admin"=w233) -> ("Addressed to this instance?"=w235:bool)  [unwired: 8 in, 1 out]
            n290 = case shown="True" w235 {
              tunnel: w233 -> [_ w237]
              frame False {
              }
              frame True {
                # "Hide the panel of this VI, and send a status updated message to let listeners know."
                n291 = property on="Property Node" class="Mod Admin"(reference=w237) -> ("Accessors:Module ID"=w236:i32)  [unwired: 1 in, 2 out]
                n292 = control-ref of="This VI"() -> (w239:refnum<vi>)
                n293 = call "Hide VI Panel.vi"("VI"=w239) -> ()  [unwired: 10 in, 1 out]
                n294 = call "Status Updated.vi"("Status"="Panel hidden." ("format string"), "Module ID"=w236) -> ()  [unwired: 9 in, 1 out]
              }
            }
          }
          event User Event {
            # "This module called the \"Private.Draw Plot\" private request."
            n295 = event-data() -> ("Module ID"=w242:i32, "布尔"=w241:bool)  [unwired: 1 in]
            n296 = Bundle(cluster=T11 {"Module ID"=-1, "布尔"=FALSE} ("Draw Plot Argument"), "Module ID"=w242, "布尔"=w241) -> (w243:T11)
            n297 = call "Addressed to This Module.vi"("Module ID from Argument"=w242, "Module Admin"=w245) -> ("Addressed to this instance?"=w246:bool)  [unwired: 8 in, 1 out]
            n298 = case "条件结构" shown="True" w246 {
              tunnel: w247 -> [_ w251]
              tunnel: w243 -> [_ w249]
              tunnel: [_ w248] -> w240
              frame False {
              }
              frame True {
                n299 = call-poly <vilib>:"Delacor_lib_QMH_Enqueue Message (poly).vi"("Message Data"=w249, "Message"="Draw Plot", "Message Queue in"=w251) -> ("error out"=w248:errorcluster)  [unwired: 7 in, 1 out]
              }
            }
          }
          event User Event {
            # "This module called the \"Private.Filte Data\" private request."
            n300 = event-data() -> ("Module ID"=w254:i32, "布尔"=w253:bool)  [unwired: 1 in]
            n301 = Bundle(cluster=T12 {"Module ID"=-1, "布尔"=FALSE} ("Filte Data Argument"), "Module ID"=w254, "布尔"=w253) -> (w255:T12)
            n302 = call "Addressed to This Module.vi"("Module ID from Argument"=w254, "Module Admin"=w257) -> ("Addressed to this instance?"=w258:bool)  [unwired: 8 in, 1 out]
            n303 = case "条件结构" shown="True" w258 {
              tunnel: w259 -> [_ w263]
              tunnel: w255 -> [_ w261]
              tunnel: [_ w260] -> w252
              frame False {
              }
              frame True {
                n304 = call-poly <vilib>:"Delacor_lib_QMH_Enqueue Message (poly).vi"("Message Data"=w261, "Message"="Filte Data", "Message Queue in"=w263) -> ("error out"=w260:errorcluster)  [unwired: 7 in, 1 out]
              }
            }
          }
          event User Event {
            # "This module called the \"Private.Menu Action\" private request."
            n305 = event-data() -> ("Module ID"=w266:i32, "项标识符"=w265:string)  [unwired: 1 in]
            n306 = Bundle(cluster=T13 {"Module ID"=-1, "项标识符"=""} ("Menu Action Argument"), "Module ID"=w266, "项标识符"=w265) -> (w267:T13)
            n307 = call "Addressed to This Module.vi"("Module ID from Argument"=w266, "Module Admin"=w269) -> ("Addressed to this instance?"=w270:bool)  [unwired: 8 in, 1 out]
            n308 = case "条件结构" shown="True" w270 {
              tunnel: w271 -> [_ w275]
              tunnel: w267 -> [_ w273]
              tunnel: [_ w272] -> w264
              frame False {
              }
              frame True {
                n309 = call-poly <vilib>:"Delacor_lib_QMH_Enqueue Message (poly).vi"("Message Data"=w273, "Message"="Menu Action", "Message Queue in"=w275) -> ("error out"=w272:errorcluster)  [unwired: 7 in, 1 out]
              }
            }
          }
          event User Event {
            # "This module called the \"Private.Open File\" private request."
            n310 = event-data() -> ("Module ID"=w278:i32, "布尔"=w277:bool)  [unwired: 1 in]
            n311 = Bundle(cluster=T14 {"Module ID"=-1, "布尔"=FALSE} ("Open File Argument"), "Module ID"=w278, "布尔"=w277) -> (w279:T14)
            n312 = call "Addressed to This Module.vi"("Module ID from Argument"=w278, "Module Admin"=w281) -> ("Addressed to this instance?"=w282:bool)  [unwired: 8 in, 1 out]
            n313 = case "条件结构" shown="True" w282 {
              tunnel: w283 -> [_ w287]
              tunnel: w279 -> [_ w285]
              tunnel: [_ w284] -> w276
              frame False {
              }
              frame True {
                n314 = call-poly <vilib>:"Delacor_lib_QMH_Enqueue Message (poly).vi"("Message Data"=w285, "Message"="Open File", "Message Queue in"=w287) -> ("error out"=w284:errorcluster)  [unwired: 7 in, 1 out]
              }
            }
          }
          event User Event {
            # "This module called the \"Private.Restore Data\" private request."
            n315 = event-data() -> ("Module ID"=w290:i32, "布尔"=w289:bool)  [unwired: 1 in]
            n316 = Bundle(cluster=T15 {"Module ID"=-1, "布尔"=FALSE} ("Restore Data Argument"), "Module ID"=w290, "布尔"=w289) -> (w291:T15)
            n317 = call "Addressed to This Module.vi"("Module ID from Argument"=w290, "Module Admin"=w293) -> ("Addressed to this instance?"=w294:bool)  [unwired: 8 in, 1 out]
            n318 = case "条件结构" shown="True" w294 {
              tunnel: w295 -> [_ w299]
              tunnel: w291 -> [_ w297]
              tunnel: [_ w296] -> w288
              frame False {
              }
              frame True {
                n319 = call-poly <vilib>:"Delacor_lib_QMH_Enqueue Message (poly).vi"("Message Data"=w297, "Message"="Restore Data", "Message Queue in"=w299) -> ("error out"=w296:errorcluster)  [unwired: 7 in, 1 out]
              }
            }
          }
          event User Event {
            # "This module called the \"Private.Set YScale\" private request."
            n320 = event-data() -> ("Module ID"=w302:i32, "布尔"=w301:bool)  [unwired: 1 in]
            n321 = Bundle(cluster=T16 {"Module ID"=-1, "布尔"=FALSE} ("Set YScale Argument"), "Module ID"=w302, "布尔"=w301) -> (w303:T16)
            n322 = call "Addressed to This Module.vi"("Module ID from Argument"=w302, "Module Admin"=w305) -> ("Addressed to this instance?"=w306:bool)  [unwired: 8 in, 1 out]
            n323 = case "条件结构" shown="True" w306 {
              tunnel: w307 -> [_ w311]
              tunnel: w303 -> [_ w309]
              tunnel: [_ w308] -> w300
              frame False {
              }
              frame True {
                n324 = call-poly <vilib>:"Delacor_lib_QMH_Enqueue Message (poly).vi"("Message Data"=w309, "Message"="Set YScale", "Message Queue in"=w311) -> ("error out"=w308:errorcluster)  [unwired: 7 in, 1 out]
              }
            }
          }
          event User Event {
            # "This module called the \"Private.Show Value\" private request."
            n325 = event-data() -> ("Module ID"=w314:i32, "坐标"=w313:T2)  [unwired: 1 in]
            n326 = Bundle(cluster=T17 {"Module ID"=-1, "坐标"={"Horizontal"=0, "Vertical"=0}} ("Show Value Argument"), "Module ID"=w314, "坐标"=w313) -> (w315:T17)
            n327 = call "Addressed to This Module.vi"("Module ID from Argument"=w314, "Module Admin"=w317) -> ("Addressed to this instance?"=w318:bool)  [unwired: 8 in, 1 out]
            n328 = case "条件结构" shown="True" w318 {
              tunnel: w319 -> [_ w323]
              tunnel: w315 -> [_ w321]
              tunnel: [_ w320] -> w312
              frame False {
              }
              frame True {
                n329 = call-poly <vilib>:"Delacor_lib_QMH_Enqueue Message (poly).vi"("Message Data"=w321, "Message"="Show Value", "Message Queue in"=w323) -> ("error out"=w320:errorcluster)  [unwired: 7 in, 1 out]
              }
            }
          }
          event User Event {
            # "This module called the \"Private.Update Curve Color\" private request."
            n330 = event-data() -> ("Module ID"=w326:i32, "布尔"=w325:bool)  [unwired: 1 in]
            n331 = Bundle(cluster=T18 {"Module ID"=-1, "布尔"=FALSE} ("Update Curve Color Argument"), "Module ID"=w326, "布尔"=w325) -> (w327:T18)
            n332 = call "Addressed to This Module.vi"("Module ID from Argument"=w326, "Module Admin"=w329) -> ("Addressed to this instance?"=w330:bool)  [unwired: 8 in, 1 out]
            n333 = case "条件结构" shown="True" w330 {
              tunnel: w331 -> [_ w335]
              tunnel: w327 -> [_ w333]
              tunnel: [_ w332] -> w324
              frame False {
              }
              frame True {
                n334 = call-poly <vilib>:"Delacor_lib_QMH_Enqueue Message (poly).vi"("Message Data"=w333, "Message"="Update Curve Color", "Message Queue in"=w335) -> ("error out"=w332:errorcluster)  [unwired: 7 in, 1 out]
              }
            }
          }
          event User Event {
            # "This module called the \"Private.Update Filter Arguments\" private request."
            n335 = event-data() -> ("Module ID"=w338:i32, "布尔"=w337:bool)  [unwired: 1 in]
            n336 = Bundle(cluster=T19 {"Module ID"=-1, "布尔"=FALSE} ("Update Filter Arguments Argument"), "Module ID"=w338, "布尔"=w337) -> (w339:T19)
            n337 = call "Addressed to This Module.vi"("Module ID from Argument"=w338, "Module Admin"=w341) -> ("Addressed to this instance?"=w342:bool)  [unwired: 8 in, 1 out]
            n338 = case "条件结构" shown="True" w342 {
              tunnel: w343 -> [_ w347]
              tunnel: w339 -> [_ w345]
              tunnel: [_ w344] -> w336
              frame False {
              }
              frame True {
                n339 = call-poly <vilib>:"Delacor_lib_QMH_Enqueue Message (poly).vi"("Message Data"=w345, "Message"="Update Filter Arguments", "Message Queue in"=w347) -> ("error out"=w344:errorcluster)  [unwired: 7 in, 1 out]
              }
            }
          }
          event User Event {
            # "This module called the \"Private.Window Resize\" private request."
            n340 = event-data() -> ("Module ID"=w350:i32, "布尔"=w349:bool)  [unwired: 1 in]
            n341 = Bundle(cluster=T20 {"Module ID"=-1, "布尔"=FALSE} ("Window Resize Argument"), "Module ID"=w350, "布尔"=w349) -> (w351:T20)
            n342 = call "Addressed to This Module.vi"("Module ID from Argument"=w350, "Module Admin"=w353) -> ("Addressed to this instance?"=w354:bool)  [unwired: 8 in, 1 out]
            n343 = case "条件结构" shown="True" w354 {
              tunnel: w355 -> [_ w359]
              tunnel: w351 -> [_ w357]
              tunnel: [_ w356] -> w348
              frame False {
              }
              frame True {
                n344 = call-poly <vilib>:"Delacor_lib_QMH_Enqueue Message (poly).vi"("Message Data"=w357, "Message"="Window Resize", "Message Queue in"=w359) -> ("error out"=w356:errorcluster)  [unwired: 7 in, 1 out]
              }
            }
          }
          event User Event {
            # "Another Module called the \"Show Diagram\" API Method. This event is used for debugging."
            n345 = event-data() -> ("Module ID"=w361:i32)  [unwired: 1 in]
            n346 = call "Addressed to This Module.vi"("Module ID from Argument"=w361, "Module Admin"=w360) -> ("Addressed to this instance?"=w362:bool)  [unwired: 8 in, 1 out]
            n347 = case shown="True" w362 {
              tunnel: w360 -> [_ w363]
              frame False {
              }
              frame True {
                n348 = disable-structure shown="RUN_TIME_ENGINE==False" {
                  disable-tunnel: w363 -> [w364 _]
                  frame condition #0 (active) {
                    # "functionality not available in exe"
                    n349 = invoke on="Invoke Node" class="VI" method="Lock State.Get"() -> (error out=w370:errorcluster, "Get Lock State"=w369:T21, "pwd in cache"=w366:bool)  [unwired: 4 in, 1 out]
                    n350 = Equal?(x=T21."Password-protected", y=w369) -> (x = y?=w367:bool)
                    n351 = Compound Arithmetic op=AND(w367, invert w366) -> (w365:bool)
                    n352 = case shown="False" w365 {
                      tunnel: w370 -> [w375 _]
                      tunnel: w364 -> [w372 _]
                      frame False {
                        n353 = property on="Property Node" class="Mod Admin"(reference=w372) -> ("Accessors:Module ID"=w371:i32)  [unwired: 1 in, 2 out]
                        n354 = property on="Property Node" class="VI"(error in=w375, "BDWin.Open"=TRUE ("Block Diagram Window:Open")) -> ()  [unwired: 1 in, 2 out]
                        n355 = call "Status Updated.vi"("Status"="Block Diagram shown." ("format string"), "Module ID"=w371) -> ()  [unwired: 9 in, 1 out]
                      }
                      frame True {
                        # "Password-protected VI, and the password is not in the cache. Do not show the diagram."
                      }
                    }
                  }
                  frame condition #1 {
                  }
                }
              }
            }
          }
          event User Event {
            # "Another Module called the \"Show Panel\" API Method."
            n356 = event-data() -> ("Module ID"=w377:i32)  [unwired: 1 in]
            n357 = call "Addressed to This Module.vi"("Module ID from Argument"=w377, "Module Admin"=w376) -> ("Addressed to this instance?"=w378:bool)  [unwired: 8 in, 1 out]
            n358 = case shown="True" w378 {
              tunnel: w376 -> [_ w380]
              frame False {
              }
              frame True {
                # "Show the panel of this VI, and send a status updated message to let listeners know."
                n359 = property on="Property Node" class="Mod Admin"(reference=w380) -> ("Accessors:Module ID"=w379:i32)  [unwired: 1 in, 2 out]
                n360 = control-ref of="This VI"() -> (w382:refnum<vi>)
                n361 = call "Open VI Panel.vi"("VI"=w382) -> ()  [unwired: 10 in, 1 out]
                n362 = call "Status Updated.vi"("Status"="Panel shown." ("format string"), "Module ID"=w379) -> ()  [unwired: 9 in, 1 out]
              }
            }
          }
          event User Event {
            # "Another Module called the \"Stop Module\" API Method  or the Message Handling Loop below."
            n363 = event-data() -> ("Module ID"=w384:i32, "Wait for Module to stop?"=w385:bool, "Origin"=w383:string)  [unwired: 1 in]
            n364 = call "Addressed to This Module.vi"("Module ID from Argument"=w384, "Module Admin"=w388) -> ("Addressed to this instance?"=w387:bool)  [unwired: 8 in, 1 out]
            n365 = case shown="True" w387 {
              tunnel: [_ w401] -> w390
              tunnel: w389 -> [_ w397]
              tunnel: [_ TRUE] -> w386
              tunnel: w385 -> [_ w392]
              tunnel: w384 -> [_ w394]
              tunnel: w383 -> [_ _]
              frame False {
              }
              frame True {
                # "The event can get fired from the Exit message. The queue gets destroyed there. In this case, the Enqueue VI will return error 1. It is safe to ignore, because the module is already exiting."
                n366 = Bundle By Name(cluster=T22 {"Module ID"=-1, "Origin"="", "Exit via Stop Module Req?"=FALSE, "Wait for Module to stop?"=FALSE} ("Stop Argument"), "Module ID"=w394, "Exit via Stop Module Req?"=TRUE, "Wait for Module to stop?"=w392) -> (w391:T22)
                n367 = call-poly <vilib>:"Delacor_lib_QMH_Enqueue Message (poly).vi"("Priority Message? (F)"=TRUE, "Message Data"=w391, "Message"="Exit", "Message Queue in"=w397) -> ("error out"=w402:errorcluster)  [unwired: 6 in, 1 out]
                n368 = call <vilib>:"Clear Errors.vi"("error in (no error)"=w402, "specific error code to clear (0: all)"=1) -> ("error out"=w401:errorcluster)  [unwired: 4 in, 1 out]
              }
            }
          }
          event Panel Resize {
            n369 = event-data() -> ()  [unwired: 1 in, 1 out]
            n370 = Enqueue Element(queue=w404, element=-1) -> ()  [unwired: 2 in, 3 out]
          }
          event Panel Close? {
            w409 = TRUE  # Discard the event, the MHL is responsible for closing and stopping this VI.
            # "Hide the panel or send the 'Exit' message if the user clicks the 'X' on the module main VI panel."
            n371 = event-data() -> ()  [unwired: 1 in, 1 out]
            n372 = property on="Property Node" class="Mod Admin" props=["Accessors:External Launch"](reference=w408) -> (reference out=w406:refnum<class "Delacor_lib_QMH_Cloneable Module Admin.lvclass">)  [unwired: 1 in, 2 out]
            n373 = case shown="True" FALSE {
              tunnel: w407 -> [_ w418]
              tunnel: [_ w419] -> w410
              tunnel: w406 -> [w413 _]
              frame True {
                # "If externally launched, clicking the 'X' hides the panel, but doesn't close it."
                n374 = property on="Property Node" class="Mod Admin"(reference=w413) -> ("Accessors:Module ID"=w412:i32)  [unwired: 1 in, 2 out]
                n375 = call "Status Updated.vi"("Status"="Panel hidden." ("format string"), "Module ID"=w412) -> ("error out"=w411:errorcluster)  [unwired: 9 in]
                n376 = control-ref of="This VI"() -> (w415:refnum<vi>)
                n377 = call "Hide VI Panel.vi"("error in"=w411, "VI"=w415) -> ()  [unwired: 9 in, 1 out]
              }
              frame False {
                # "If run as a stand-alone VI, clicking the panel 'X' stops the VI."
                n378 = call-poly <vilib>:"Delacor_lib_QMH_Enqueue Message (poly).vi"("Priority Message? (F)"=TRUE, "Message"="Exit", "Message Queue in"=w418) -> ("error out"=w419:errorcluster)  [unwired: 7 in, 1 out]
              }
            }
            n379 = event-data ("Event Filter Node")("Discard?"=w409) -> ()  [unwired: 1 in, 1 out]
          }
          event User Event {
            # "This module called the \"Private.Cut Half Data\" private request."
            n380 = event-data() -> ("Module ID"=w422:i32, "布尔"=w421:bool)  [unwired: 1 in]
            n381 = Bundle(cluster=T23 {"Module ID"=-1, "布尔"=FALSE} ("Cut Half Data Argument"), "Module ID"=w422, "布尔"=w421) -> (w423:T23)
            n382 = call "Addressed to This Module.vi"("Module ID from Argument"=w422, "Module Admin"=w425) -> ("Addressed to this instance?"=w426:bool)  [unwired: 8 in, 1 out]
            n383 = case "条件结构" shown="True" w426 {
              tunnel: w427 -> [_ w431]
              tunnel: w423 -> [_ w429]
              tunnel: [_ w428] -> w420
              frame False {
              }
              frame True {
                n384 = call-poly <vilib>:"Delacor_lib_QMH_Enqueue Message (poly).vi"("Message Data"=w429, "Message"="Cut Half Data", "Message Queue in"=w431) -> ("error out"=w428:errorcluster)  [unwired: 7 in, 1 out]
              }
            }
          }
          event User Event {
            # "Another Module called the \"Scale List Menu Action\" API Method."
            n385 = event-data() -> ("Module ID"=w435:i32, "ItemTag"=w434:string, "Scale Index"=w433:i32)  [unwired: 1 in]
            n386 = Bundle(cluster=T24 {"Module ID"=-1, "ItemTag "="", "Scale Index"=0} ("Scale List Menu Action Argument"), "Module ID"=w435, "ItemTag"=w434, "Scale Index"=w433) -> (w436:T24)
            n387 = call "Addressed to This Module.vi"("Module ID from Argument"=w435, "Module Admin"=w438) -> ("Addressed to this instance?"=w439:bool)  [unwired: 8 in, 1 out]
            n388 = case shown="True" w439 {
              tunnel: w440 -> [_ w444]
              tunnel: w436 -> [_ w442]
              tunnel: [_ w441] -> w432
              frame False {
              }
              frame True {
                n389 = call-poly <vilib>:"Delacor_lib_QMH_Enqueue Message (poly).vi"("Message Data"=w442, "Message"="Scale List Menu Action", "Message Queue in"=w444) -> ("error out"=w441:errorcluster)  [unwired: 7 in, 1 out]
              }
            }
          }
          event User Event {
            # "This module called the \"Private.Update Scale List\" private request."
            n390 = event-data() -> ("Module ID"=w447:i32, "Boolean"=w446:bool)  [unwired: 1 in]
            n391 = Bundle(cluster=T25 {"Module ID"=-1, "Boolean"=FALSE} ("Update Scale List Argument"), "Module ID"=w447, "Boolean"=w446) -> (w448:T25)
            n392 = call "Addressed to This Module.vi"("Module ID from Argument"=w447, "Module Admin"=w450) -> ("Addressed to this instance?"=w451:bool)  [unwired: 8 in, 1 out]
            n393 = case shown="True" w451 {
              tunnel: w452 -> [_ w456]
              tunnel: w448 -> [_ w454]
              tunnel: [_ w453] -> w445
              frame False {
              }
              frame True {
                n394 = call-poly <vilib>:"Delacor_lib_QMH_Enqueue Message (poly).vi"("Message Data"=w454, "Message"="Update Scale List", "Message Queue in"=w456) -> ("error out"=w453:errorcluster)  [unwired: 7 in, 1 out]
              }
            }
          }
          event User Event {
            # "This module called the \"Private.Initialize Plot List\" private request."
            n395 = event-data() -> ("Module ID"=w459:i32, "Boolean"=w458:bool)  [unwired: 1 in]
            n396 = Bundle(cluster=T26 {"Module ID"=-1, "Boolean"=FALSE} ("Initialize Plot List Argument"), "Module ID"=w459, "Boolean"=w458) -> (w460:T26)
            n397 = call "Addressed to This Module.vi"("Module ID from Argument"=w459, "Module Admin"=w462) -> ("Addressed to this instance?"=w463:bool)  [unwired: 8 in, 1 out]
            n398 = case shown="True" w463 {
              tunnel: w464 -> [_ w468]
              tunnel: w460 -> [_ w466]
              tunnel: [_ w465] -> w457
              frame False {
              }
              frame True {
                n399 = call-poly <vilib>:"Delacor_lib_QMH_Enqueue Message (poly).vi"("Message Data"=w466, "Message"="Initialize Plot List", "Message Queue in"=w468) -> ("error out"=w465:errorcluster)  [unwired: 7 in, 1 out]
              }
            }
          }
          event User Event {
            # "This module called the \"Private.Load Plot\" private request."
            n400 = event-data() -> ("Module ID"=w471:i32, "Plot Index"=w470:i32)  [unwired: 1 in]
            n401 = Bundle(cluster=T27 {"Module ID"=-1, "Plot Index"=0} ("Load Plot Argument"), "Module ID"=w471, "Plot Index"=w470) -> (w472:T27)
            n402 = call "Addressed to This Module.vi"("Module ID from Argument"=w471, "Module Admin"=w474) -> ("Addressed to this instance?"=w475:bool)  [unwired: 8 in, 1 out]
            n403 = case shown="True" w475 {
              tunnel: w476 -> [_ w480]
              tunnel: w472 -> [_ w478]
              tunnel: [_ w477] -> w469
              frame False {
              }
              frame True {
                n404 = call-poly <vilib>:"Delacor_lib_QMH_Enqueue Message (poly).vi"("Message Data"=w478, "Message"="Load Plot", "Message Queue in"=w480) -> ("error out"=w477:errorcluster)  [unwired: 7 in, 1 out]
              }
            }
          }
          event User Event {
            # "This module called the \"Private.Unload Plot\" private request."
            n405 = event-data() -> ("Module ID"=w483:i32, "Plot Index"=w482:i32)  [unwired: 1 in]
            n406 = Bundle(cluster=T28 {"Module ID"=-1, "Plot Index"=0} ("Unload Plot Argument"), "Module ID"=w483, "Plot Index"=w482) -> (w484:T28)
            n407 = call "Addressed to This Module.vi"("Module ID from Argument"=w483, "Module Admin"=w486) -> ("Addressed to this instance?"=w487:bool)  [unwired: 8 in, 1 out]
            n408 = case shown="True" w487 {
              tunnel: w488 -> [_ w492]
              tunnel: w484 -> [_ w490]
              tunnel: [_ w489] -> w481
              frame False {
              }
              frame True {
                n409 = call-poly <vilib>:"Delacor_lib_QMH_Enqueue Message (poly).vi"("Message Data"=w490, "Message"="Unload Plot", "Message Queue in"=w492) -> ("error out"=w489:errorcluster)  [unwired: 7 in, 1 out]
              }
            }
          }
          event User Event {
            # "Another Module called the \"Show Hide Scale\" API Method."
            n410 = event-data() -> ("Module ID"=w496:i32, "Scale Index"=w495:i32, "Visible"=w494:bool)  [unwired: 1 in]
            n411 = Bundle(cluster=T29 {"Module ID"=-1, "Scale Index"=0, "Visible"=FALSE} ("Show Hide Scale Argument"), "Module ID"=w496, "Scale Index"=w495, "Visible"=w494) -> (w497:T29)
            n412 = call "Addressed to This Module.vi"("Module ID from Argument"=w496, "Module Admin"=w499) -> ("Addressed to this instance?"=w500:bool)  [unwired: 8 in, 1 out]
            n413 = case shown="True" w500 {
              tunnel: w501 -> [_ w505]
              tunnel: w497 -> [_ w503]
              tunnel: [_ w502] -> w493
              frame False {
              }
              frame True {
                n414 = call-poly <vilib>:"Delacor_lib_QMH_Enqueue Message (poly).vi"("Message Data"=w503, "Message"="Show Hide Scale", "Message Queue in"=w505) -> ("error out"=w502:errorcluster)  [unwired: 7 in, 1 out]
              }
            }
          }
          event User Event {
            # "This module called the \"Private.Add Default Scale\" private request."
            n415 = event-data() -> ("Module ID"=w508:i32, "Boolean"=w507:bool)  [unwired: 1 in]
            n416 = Bundle(cluster=T30 {"Module ID"=-1, "Boolean"=FALSE} ("Add Default Scale Argument"), "Module ID"=w508, "Boolean"=w507) -> (w509:T30)
            n417 = call "Addressed to This Module.vi"("Module ID from Argument"=w508, "Module Admin"=w511) -> ("Addressed to this instance?"=w512:bool)  [unwired: 8 in, 1 out]
            n418 = case shown="True" w512 {
              tunnel: w513 -> [_ w517]
              tunnel: w509 -> [_ w515]
              tunnel: [_ w514] -> w506
              frame False {
              }
              frame True {
                n419 = call-poly <vilib>:"Delacor_lib_QMH_Enqueue Message (poly).vi"("Message Data"=w515, "Message"="Add Default Scale", "Message Queue in"=w517) -> ("error out"=w514:errorcluster)  [unwired: 7 in, 1 out]
              }
            }
          }
          event User Event {
            # "This module called the \"Private.Update Plot List\" private request."
            n420 = event-data() -> ("Module ID"=w520:i32, "曲线列表"=w519:T7)  [unwired: 1 in]
            n421 = Bundle(cluster=T31 {"Module ID"=-1, "曲线列表"=[]} ("Update Plot List Argument"), "Module ID"=w520, "曲线列表"=w519) -> (w521:T31)
            n422 = call "Addressed to This Module.vi"("Module ID from Argument"=w520, "Module Admin"=w523) -> ("Addressed to this instance?"=w524:bool)  [unwired: 8 in, 1 out]
            n423 = case shown="True" w524 {
              tunnel: w525 -> [_ w529]
              tunnel: w521 -> [_ w527]
              tunnel: [_ w526] -> w518
              frame False {
              }
              frame True {
                n424 = call-poly <vilib>:"Delacor_lib_QMH_Enqueue Message (poly).vi"("Message Data"=w527, "Message"="Update Plot List", "Message Queue in"=w529) -> ("error out"=w526:errorcluster)  [unwired: 7 in, 1 out]
              }
            }
          }
          event User Event {
            # "This module called the \"Private.Add Virtual Cruve\" private request."
            n425 = event-data() -> ("Module ID"=w532:i32, "Boolean"=w531:bool)  [unwired: 1 in]
            n426 = Bundle(cluster=T32 {"Module ID"=-1, "Boolean"=FALSE} ("Add Virtual Cruve Argument"), "Module ID"=w532, "Boolean"=w531) -> (w533:T32)
            n427 = call "Addressed to This Module.vi"("Module ID from Argument"=w532, "Module Admin"=w535) -> ("Addressed to this instance?"=w536:bool)  [unwired: 8 in, 1 out]
            n428 = case shown="True" w536 {
              tunnel: w537 -> [_ w541]
              tunnel: w533 -> [_ w539]
              tunnel: [_ w538] -> w530
              frame False {
              }
              frame True {
                n429 = call-poly <vilib>:"Delacor_lib_QMH_Enqueue Message (poly).vi"("Message Data"=w539, "Message"="Add Virtual Cruve", "Message Queue in"=w541) -> ("error out"=w538:errorcluster)  [unwired: 7 in, 1 out]
              }
            }
          }
          event User Event {
            # "This module called the \"Private.Edit Curve\" private request."
            n430 = event-data() -> ("Module ID"=w544:i32, "Plot Index"=w543:i32)  [unwired: 1 in]
            n431 = Bundle(cluster=T33 {"Module ID"=-1, "Plot Index"=0} ("Edit Curve Argument"), "Module ID"=w544, "Plot Index"=w543) -> (w545:T33)
            n432 = call "Addressed to This Module.vi"("Module ID from Argument"=w544, "Module Admin"=w547) -> ("Addressed to this instance?"=w548:bool)  [unwired: 8 in, 1 out]
            n433 = case shown="True" w548 {
              tunnel: w549 -> [_ w553]
              tunnel: w545 -> [_ w551]
              tunnel: [_ w550] -> w542
              frame False {
              }
              frame True {
                n434 = call-poly <vilib>:"Delacor_lib_QMH_Enqueue Message (poly).vi"("Message Data"=w551, "Message"="Edit Curve", "Message Queue in"=w553) -> ("error out"=w550:errorcluster)  [unwired: 7 in, 1 out]
              }
            }
          }
        }
        n435 = call-dynamic "Delacor_lib_QMH_Error Handler - Event Handling Loop.vi"("error in"=w125, "Message Queue in"=w120) -> ("dup error in"=w124:errorcluster)  [unwired: 8 in, 1 out]
      }
      n436 = while {
        tunnel: w65 -> [w82]
        tunnel: w64 -> [w79]
        stop <- w81 stop-if-true
        # "多击及延时处理"
        n437 = property class="Mod Admin"(reference=w79) -> ("Accessors:Module ID"=w78:i32)  [unwired: 1 in, 2 out]
        n438 = Dequeue Element(queue=w82) -> (queue out=w80:refnum<queue>, element=w77:i32, error out=w81:errorcluster)  [unwired: 2 in, 1 out]
        n439 = case shown="0, Default" w77 {
          selector: w77 -> [w83 _ _]
          tunnel: w80 -> [w88 w103 w111]
          tunnel: w78 -> [w84 w102 w110]
          frame 0, Default {
            n440 = while {
              tunnel: w88 -> [w99]
              tunnel: [w97] -> w87
              tunnel: [w96] -> w86
              i -> [w96]
              stop <- w95 stop-if-true
              n441 = Dequeue Element(queue=w99, timeout in ms (-1)=350) -> (queue out=w97:refnum<queue>, timed out?=w95:bool)  [unwired: 1 in, 2 out]
            }
            n442 = Increment(x=w86) -> (x+1=w85:i32)
            n443 = Flush Queue(queue=w87) -> ()  [unwired: 1 in, 3 out]
            n444 = case shown="4" w85 {
              tunnel: w83 -> [_ w89 w91 w93]
              tunnel: w84 -> [_ w90 w92 w94]
              frame 0, Default {
              }
              frame 2 {
                n445 = call "Load Plot.vi"("Plot Index"=w89, "Module ID"=w90) -> ()  [unwired: 9 in, 1 out]
              }
              frame 3 {
                n446 = call "Edit Curve.vi"("Plot Index"=w91, "Module ID"=w92) -> ()  [unwired: 9 in, 1 out]
              }
              frame 4 {
                n447 = call "Unload Plot.vi"("Plot Index"=w93, "Module ID"=w94) -> ()  [unwired: 9 in, 1 out]
              }
            }
          }
          frame -2 {
            n448 = while {
              tunnel: w103 -> [w108]
              tunnel: [w106] -> w104
              stop <- w105 stop-if-true
              n449 = Dequeue Element(queue=w108, timeout in ms (-1)=20) -> (queue out=w106:refnum<queue>, timed out?=w105:bool)  [unwired: 1 in, 2 out]
            }
            n450 = local read "Coords"() -> (w100:T2)
            n451 = Flush Queue(queue=w104) -> (error out=w101:errorcluster)  [unwired: 1 in, 2 out]
            n452 = call "Show Value.vi"("error in"=w101, "坐标"=w100, "Module ID"=w102) -> ()  [unwired: 8 in, 1 out]
          }
          frame -1 {
            # "针对窗口大小改变的延时处理，只有在窗口大小在250ms内不再改变时，才执行相应的改变控件大小的操作"
            n453 = while {
              tunnel: w111 -> [w116]
              tunnel: [w114] -> w112
              stop <- w113 stop-if-true
              n454 = Dequeue Element(queue=w116, timeout in ms (-1)=250) -> (queue out=w114:refnum<queue>, timed out?=w113:bool)  [unwired: 1 in, 2 out]
            }
            n455 = Flush Queue(queue=w112) -> (error out=w109:errorcluster)  [unwired: 1 in, 2 out]
            n456 = call "Window Resize.vi"("error in"=w109, "Module ID"=w110) -> ()  [unwired: 9 in, 1 out]
          }
        }
      }
    }
    frame Error {
      n457 = call "Synchronize Caller Events.vi"("Module Admin"=w941) -> ("Module Admin out"=w940:refnum<class "Delacor_lib_QMH_Cloneable Module Admin.lvclass">)  [unwired: 9 in, 1 out]
      n458 = property on="Property Node" class="Mod Admin"(reference=w940) -> ("Accessors:Module ID"=w939:i32)  [unwired: 1 in, 2 out]
      n459 = call-dynamic "Delacor_lib_QMH_Release Message Queue.vi"("error in"=w947, "Message Queue"=w938) -> ("error out"=w946:errorcluster)  [unwired: 9 in]
      n460 = call "Module Name--constant.vi"("Module ID"=w939) -> ("Module Name"=w944:string)  [unwired: 10 in]
      n461 = Format Into String(format string="An error occurred during initialization. %s is no longer running.", w944) -> (resulting string=w942:string)  [unwired: 2 in, 1 out]
      n462 = call "Error Reported.vi"("Additional Information"=w942, "Error"=w946, "Module ID"=w939) -> ()  [unwired: 8 in, 1 out]
    }
  }
  n463 = Merge Errors(w55, w35, w54) -> (w56:errorcluster)
  n464 = call "Close Module.vi"("error in"=w56, "Wait for stop?"=w43, "Module Admin in"=w25) -> ("error out"=w52:errorcluster, "External Launch"=w42:bool, "Module Admin out"=w44:refnum<class "Delacor_lib_QMH_Cloneable Module Admin.lvclass">)  [unwired: 6 in]
  n465 = Unregister For Events(event registration refnum=w49, error in=w52) -> (error out=w9:errorcluster)
  "错误输出" <- w9
  n466 = local write "Module Admin"(w44) -> ()
  n467 = case "External Launch?" shown="True" w42 {
    tunnel: w9 -> [_ w948]
    frame False {
    }
    frame True {
      n468 = case shown="No Error" w948 {
        frame No Error {
          n469 = invoke class="VI" method="FP.Close"() -> ()  [unwired: 3 in, 3 out]
        }
        frame Error {
          n470 = invoke class="VI" method="FP.Open"("Activate"=TRUE ("Activate?")) -> ()  [unwired: 4 in, 5 out]
        }
      }
    }
  }
  n471 = call <vilib>:"Clear Errors.vi"("error in (no error)"=w9) -> ("error out"=w7:errorcluster)  [unwired: 5 in, 1 out]
  n472 = property class="App"(error in=w7) -> ("App.Kind"=w8:T39)  [unwired: 1 in, 2 out]
  n473 = case shown="\"Run Time System\"" w8 {
    frame "Development System", Default {
    }
    frame "Run Time System" {
      n474 = invoke class="VI" method="FP.Close"() -> ()  [unwired: 3 in, 3 out]
    }
  }
  "XY图" <- cluster{"Time":timestamp[], "Value":dbl[]}[] []
